vi "Main.vi"(11 "Module Admin":refnum<class "Delacor_lib_QMH_Module Admin.lvclass">) -> ()   [LabVIEW 2025, in "Auto-Process.lvlib"]
doc: "This template is based off of the Queued Message Handler design pattern and the Queued Message Handler project template that ships with LabVIEW.\n\nThe main difference is that the queue is private to this module and communication between modules is performed via Broadcast and Request events.\n\nRequest events are wrapped in public API methods and are handled in the Event Handling Loop (EHL) of this VI. Any module can register for Broadcast events sent by this module. The EHL generates messages based on user interface actions.\n\nThe Message Handling Loop (MHL) processes messages generated by the EHL, or by other messages. The messages are string values, so new messages can be added easily to the Message Cases case structure in the MHL. Each message cluster can also provide an optional value for Message Data, which is a variant that can be converted to whatever message-specific data is required.\n_____\nBased on DQMH Dev Tools: Project Template 7.1.1.1528."
uses:
  Auto-Process.lvlib
  <vilib>/Delacor/Delacor QMH/Libraries/Module Admin_class/Delacor_lib_QMH_Module Admin.lvclass
  Subvi-G/Control/XButton/button3.xctl
  <vilib>/Utility/miscctls.llb/LVPointTypeDef.ctl
  <vilib>/Utility/miscctls.llb/LVPositionTypeDef.ctl
  Module Data--cluster.ctl
  Database/Database_access.lvclass
  Do Something Argument--cluster.ctl
  <vilib>/Delacor/Delacor QMH/Libraries/Message Queue_class/Delacor_lib_QMH_Message Queue.lvclass/Delacor_lib_QMH_Message Queue.ctl
  Do Something Else Argument--cluster.ctl
  Do Something Else and Wait for Reply Argument--cluster.ctl
  Do Something Else and Wait (Reply Payload)--cluster.ctl
  Stop Argument--cluster.ctl
  <vilib>/Delacor/Delacor QMH/Libraries/Module Admin_class/Delacor_lib_QMH_Module Admin.lvclass/Delacor_lib_QMH_Module Admin.ctl
  Edit.ctl
  Origin Argument--cluster.ctl
  Init-External Argument--cluster.ctl
  Requst Execution Status Argument--cluster.ctl
  Requst Execution Status (Reply Payload)--cluster.ctl
  Receive end Argument--cluster.ctl
  <vilib>/Utility/miscctls.llb/LVBoundsTypeDef.ctl
  Database/Son-control.ctl
  <vilib>/addons/database/Auxilliary.llb/DB Tools Column Info.ctl
  <vilib>/addons/database/Auxilliary.llb/DB Tools DataTypes.ctl
  <vilib>/Delacor/Delacor QMH/Libraries/Message Queue_class/Delacor_lib_QMH_Enqueue Message (Single).vi
  <vilib>/Delacor/Delacor QMH/Libraries/Module Admin_class/Delacor_lib_QMH_Get External Launch.vi
  <vilib>/Delacor/Delacor QMH/Libraries/Message Queue_class/Delacor_lib_QMH_Enqueue Message (Array).vi
  <vilib>/Delacor/Delacor QMH/Libraries/Message Queue_class/Delacor_lib_QMH_Message Queue.lvclass
  <vilib>/addons/database/NI_Database_API.lvlib
panel:
  in  "窗口标题":string
  out "Business rule":string
  in  "Valued":string
  in  "Combo Box":string(combo)
  in  "Edit?":bool
  in  "返回主界面":bool(xcontrol)
  in  "编辑显示退表":i32[](listbox)
  in  "编辑显示进表":i32[](listbox)
  in  "编辑显示总览":i32[](listbox)
  in  "结束":bool(xcontrol)
  in  "暂停":bool(xcontrol)
  in  "开始":bool(xcontrol)
  out "logging":string
  in  "执行显示":i32[](listbox)
  in  "任务显示":i32[](listbox)
  out "error out":errorcluster
  out "X":dbl
  out "Status":string
  in  "Simulate MHL Error":bool
  in  "Simulate EHL Error":bool
  in  "Do Something Else <Replace Me>":bool
  in  "Do Something <Replace Me>":bool
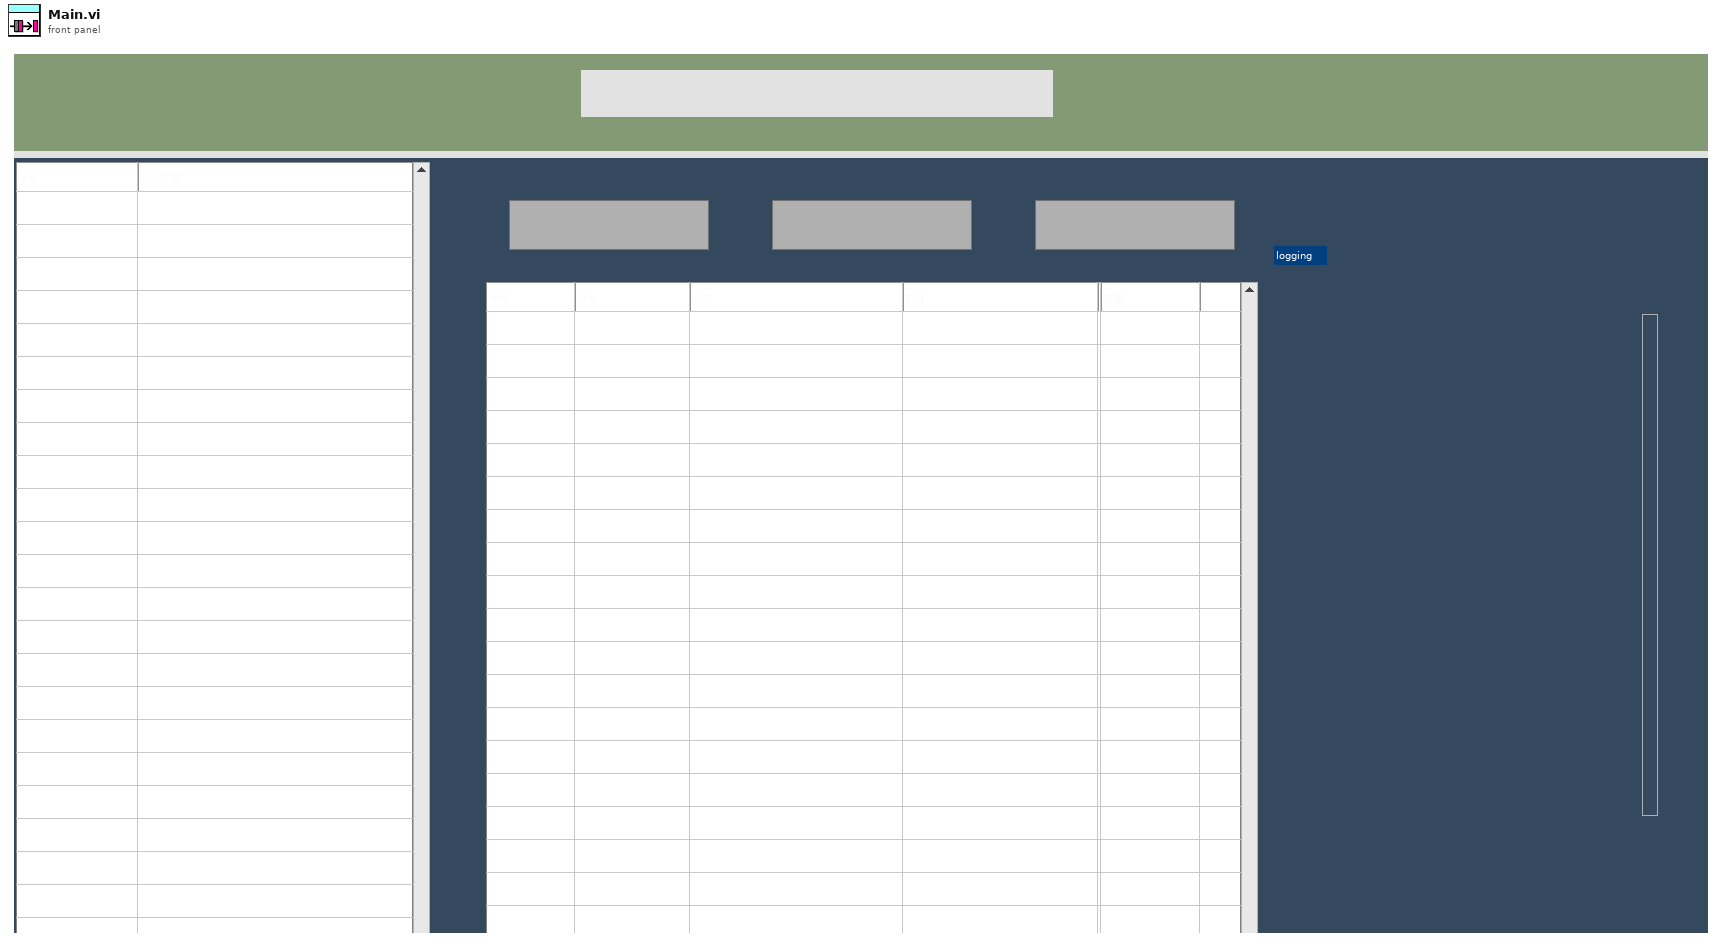
[diagram p1: front panel]
types:
  T1 = typedef "LVPositionTypeDef.ctl" = cluster{"Left":i32, "Top":i32}
  T2 = typedef "LVPointTypeDef.ctl" = cluster{"Horizontal":i16, "Vertical":i16}
  T3 = typedef "Auto-Process.lvlib/Request Events--cluster.ctl" = cluster{"Stop Module":refnum<user-event>, "Do Something":refnum<user-event>, "Do Something Else":refnum<user-event>, "Do Something Else and Wait for Reply":refnum<user-event>, "Show Panel":refnum<user-event>, "Hide Panel":refnum<user-event>, "Get Module Execution Status":refnum<user-event>, "Show Diagram":refnum<user-event>, "Origin":refnum<user-event>, "Init-External":refnum<user-event>, "Requst Execution Status":refnum<user-event>, "Receive end":refnum<user-event>, "Refursh-UI":refnum<user-event>}
  T4 = typedef "Auto-Process.lvlib/Module Data--cluster.ctl" = cluster{"Status":string, "Databas":refnum<class "Database_access.lvclass">, "总览表寄存器":string[][], "总览大小":i32[], "动作":string[][], "行为":string[], "数据类型":string[], "进表寄存器":string[][], "退表寄存器":string[][], "进退自如":u8, "选择表名":string, "New-table":string, "Old-table":string, "进退自如":bool, "行列号":cluster{"Row":i32, "Column":i32}, "项符号":i32[], "Choosed task":string[], "Remaining table":string[], "Remaining Process":string[][], "Execute Process":string[][], "暂停指令":string}
  T5 = typedef "Auto-Process.lvlib/Do Something Argument--cluster.ctl" = cluster{"Do Something Msg":string}
  T6 = typedef "Auto-Process.lvlib/Do Something Else Argument--cluster.ctl" = cluster{"Do Something Else Msg":string, "X":dbl}
  T7 = typedef "Auto-Process.lvlib/Do Something Else and Wait for Reply Argument--cluster.ctl" = cluster{"Do Something Else Msg":string, "X":dbl, "Wait Notifier":refnum<notifier>, "wait for reply":bool}
  T8 = enum32{"invalid lock state", "Not Locked", "Locked (No Password)", "Password-protected"}
  T9 = typedef "Auto-Process.lvlib/Stop Argument--cluster.ctl" = cluster{"Origin":string, "Exit via Stop Module Req?":bool, "Wait for Module to stop?":bool}
  T10 = typedef "Edit.ctl" = cluster{"单元格位置":cluster{"Row":i32, "Column":i32}, "控件引用":refnum<vi>, "进退自如":u8}
  T11 = typedef "Auto-Process.lvlib/Origin Argument--cluster.ctl" = cluster{"原点":cluster{"Horizontal":i16, "Vertical":i16}}
  T12 = typedef "Auto-Process.lvlib/Init-External Argument--cluster.ctl" = cluster{"布尔":bool}
  T13 = typedef "Auto-Process.lvlib/Requst Execution Status Argument--cluster.ctl" = cluster{"Wait Notifier":refnum<notifier>, "wait for reply":bool}
  T14 = typedef "Auto-Process.lvlib/Receive end Argument--cluster.ctl" = cluster{"Arr":string[]}
  T15 = enum32{"Invalid", "Standard", "Closed", "Hidden", "Minimized", "Maximized"}
  T16 = enum8{"Enabled", "Disabled", "Disabled and Grayed Out"}
  T17 = typedef "Auto-Process.lvlib/Do Something Else and Wait (Reply Payload)--cluster.ctl" = cluster{"Value":dbl, "error":errorcluster}
  T18 = typedef "Auto-Process.lvlib/Requst Execution Status (Reply Payload)--cluster.ctl" = cluster{"Status":enum8{"Enabled", "Disabled", "Disabled and Grayed Out"}, "error":errorcluster}
  T19 = typedef "LVBoundsTypeDef.ctl" = cluster{"Width":u32, "Height":u32}
  T20 = cluster{"退表寄存器[0]":string, "退表寄存器[1]":string, "退表寄存器[2]":string, "退表寄存器[3]":string, "退表寄存器[4]":string}
  T21 = cluster{"字符串":string, "字符串 2":string, "字符串 3":string, "字符串 4":string, "字符串 5":string}
  T22 = typedef "Son-control.ctl" = T23[]
  T23 = typedef "NI_Database_API.lvlib/DB Tools Column Info.ctl" = cluster{"column name":string, "data type":T24, "size":i32, "allow null?":bool}
  T24 = typedef "NI_Database_API.lvlib/DB Tools DataTypes.ctl" = enum16{"String", "Long (I32)", "Single (SGL)", "Double (DBL)", "Date/Time", "Binary"}
  T25 = cluster{"总览表寄存器[0]":string, "总览表寄存器[1]":string, "总览表寄存器[2]":string}
  T26 = typedef "LVPoint32TypeDef.ctl" = cluster{"Horizontal":i32, "Vertical":i32}
  T27 = typedef "LVRowAndColumnTypeDef.ctl" = cluster{"Row":i32, "Column":i32}
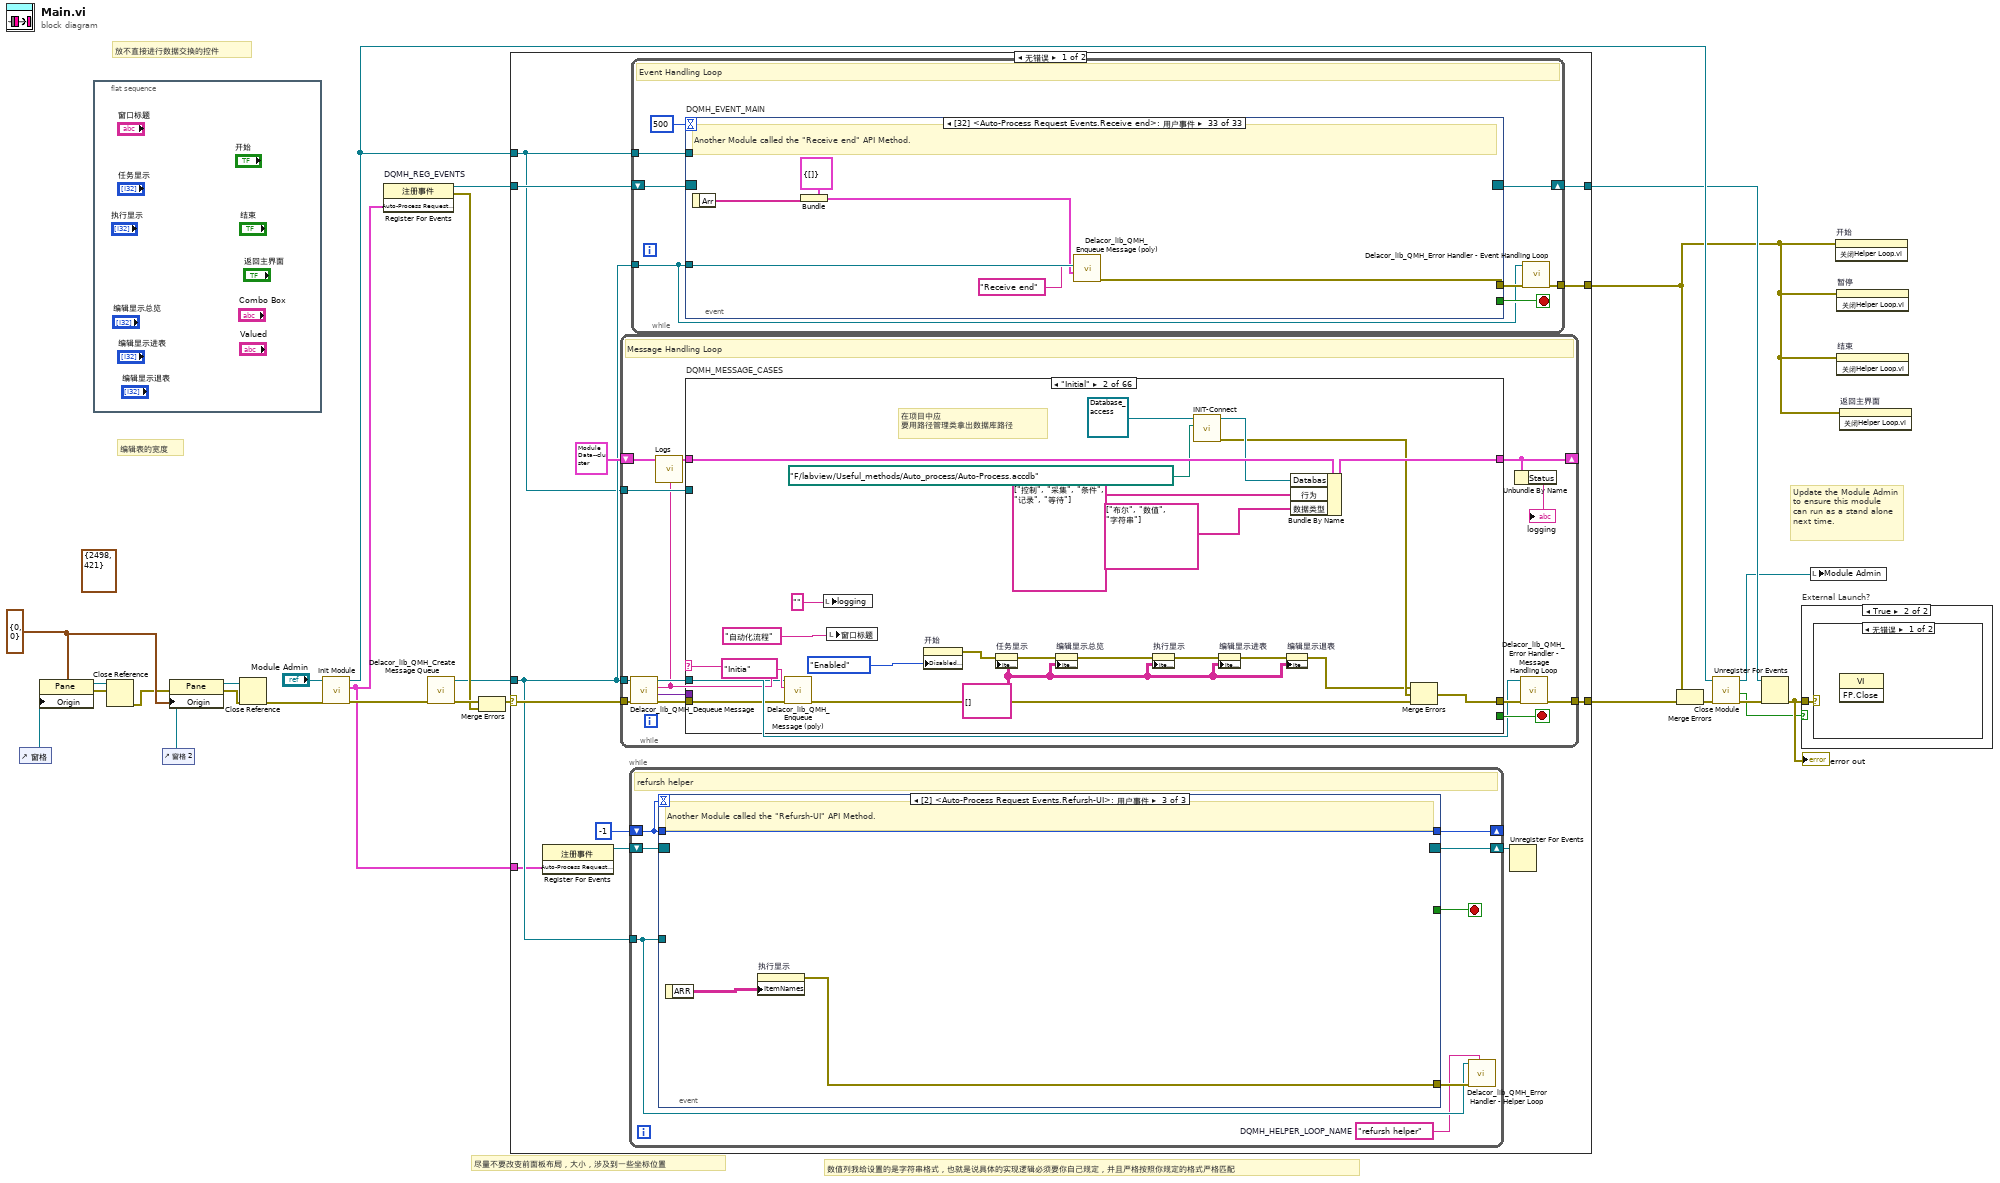
[diagram p0: block diagram]
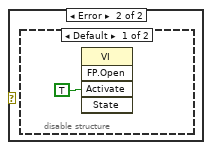
[diagram p3: hidden frame]
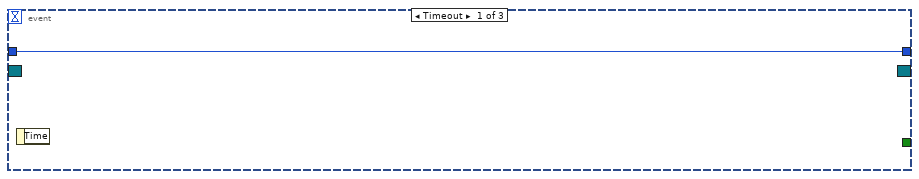
[diagram p5: hidden frame]
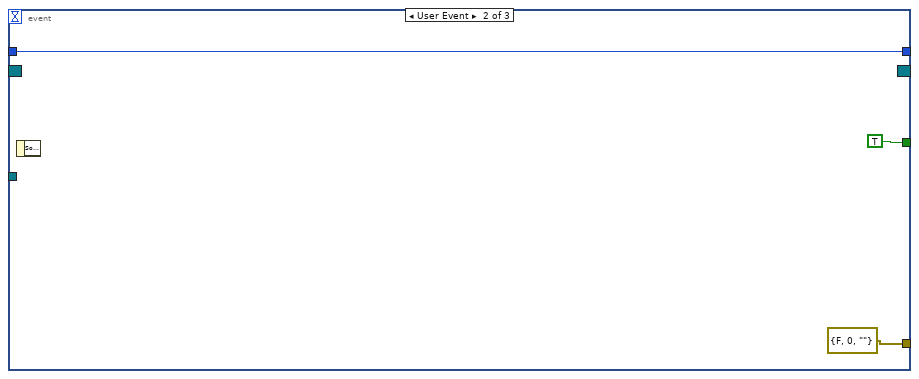
[diagram p6: hidden frame]
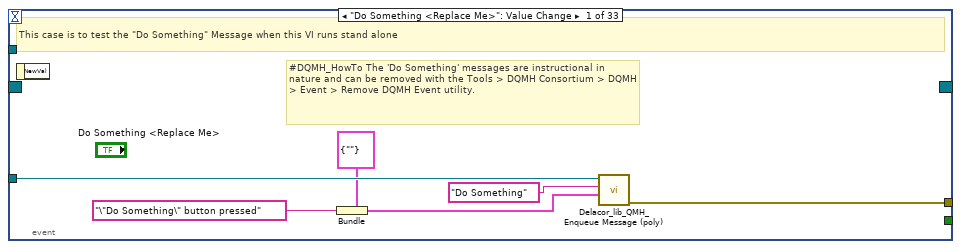
[diagram p7: hidden frame]
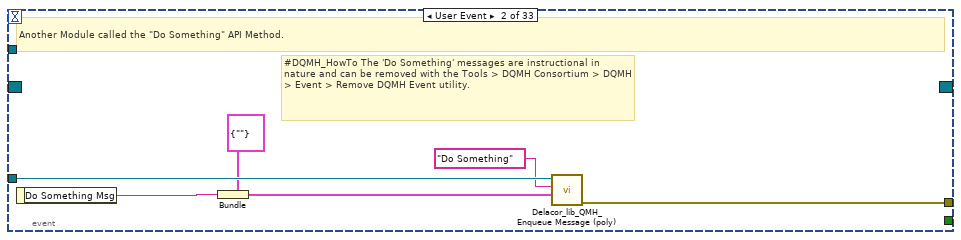
[diagram p8: hidden frame]
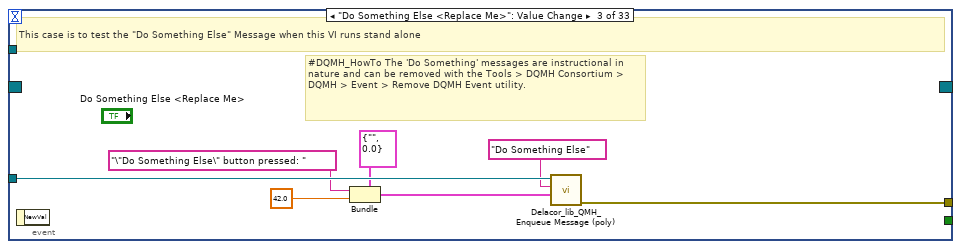
[diagram p9: hidden frame]
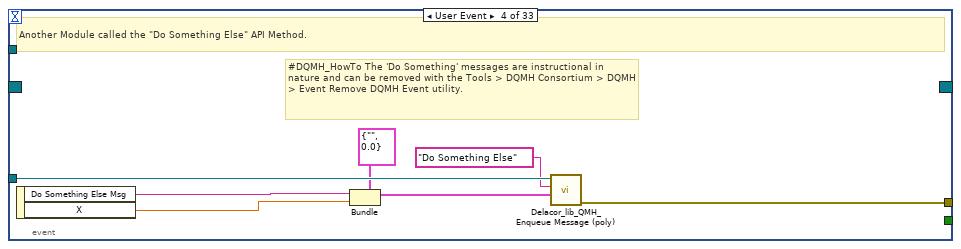
[diagram p10: hidden frame]
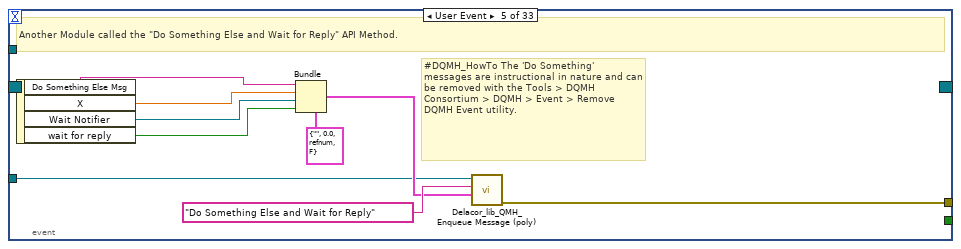
[diagram p11: hidden frame]
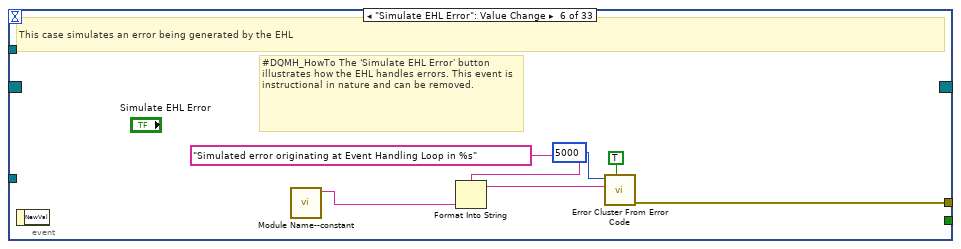
[diagram p12: hidden frame]
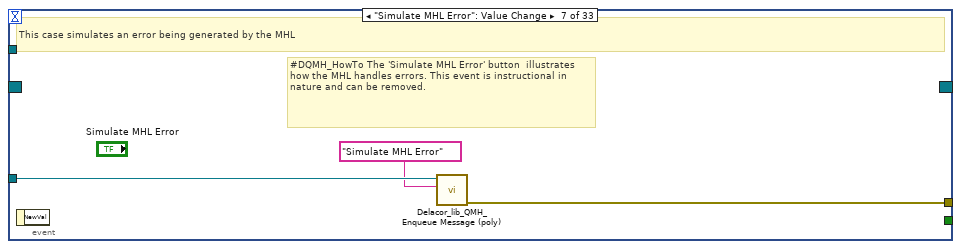
[diagram p13: hidden frame]
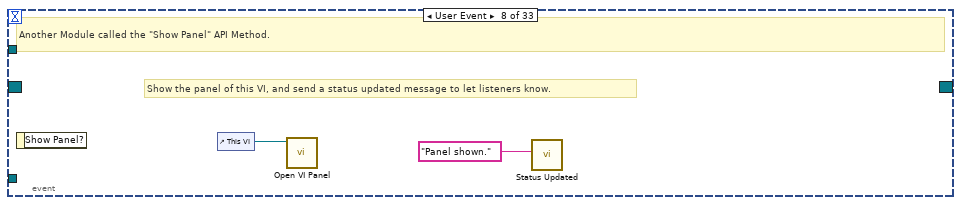
[diagram p14: hidden frame]
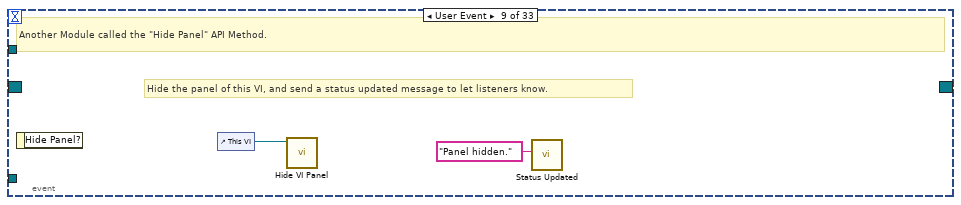
[diagram p15: hidden frame]
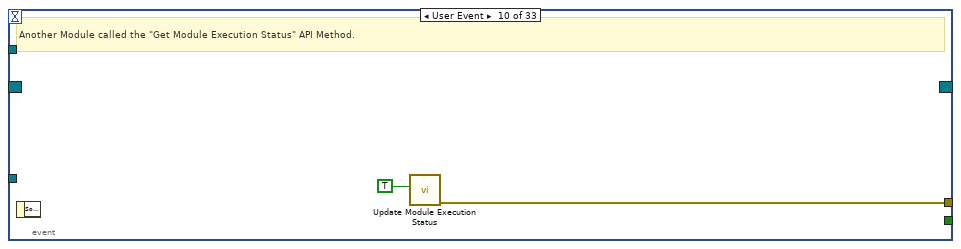
[diagram p16: hidden frame]
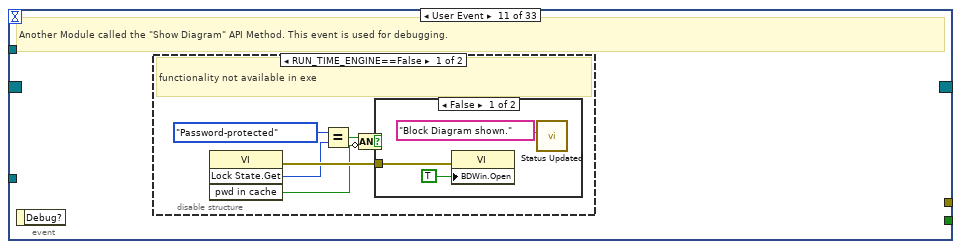
[diagram p17: hidden frame]
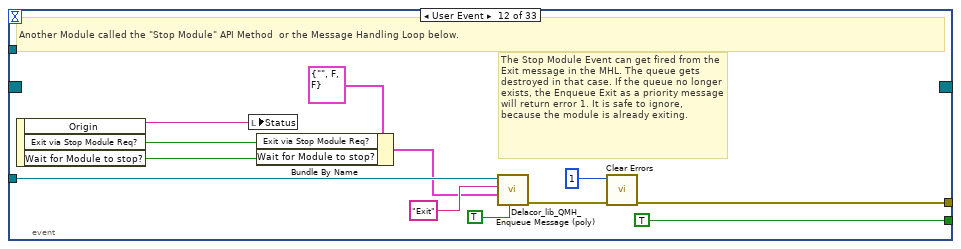
[diagram p20: hidden frame]
diagram:
  (unwired) T1 {"Left"=2498, "Top"=421} ("位置 2")
  w9 = T2 {"Horizontal"=0, "Vertical"=0} ("原点")
  # "数值列我给设置的是字符串格式，也就是说具体的实现逻辑必须要你自己规定，并且严格按照你规定的格式严格匹配"
  # "尽量不要改变前面板布局，大小，涉及到一些坐标位置"
  # "编辑表的宽度"
  # "放不直接进行数据交换的控件"
  # "Update the Module Admin to ensure this module can run as a stand alone next time."
  n1 = control-ref of="窗格"() -> (w11:refnum<vi>)
  n2 = property class="Pane"(reference=w11, "Origin"=w9) -> (reference out=w5:refnum<vi>, error out=w6:errorcluster)  [unwired: 1 in]
  n3 = flat-sequence {
    frame #0 {
    }
  }
  n4 = Close Reference(reference=w5, error in (no error)=w6) -> (error out=w4:errorcluster)
  n5 = control-ref of="窗格 2"() -> (w10:refnum<vi>)
  n6 = property class="Pane"(reference=w10, error in=w4, "Origin"=w9) -> (reference out=w7:refnum<vi>, error out=w8:errorcluster)
  n7 = Close Reference(reference=w7, error in (no error)=w8) -> (error out=w3:errorcluster)
  n8 = call "Init Module.vi"("error in"=w3, "Singleton Module Admin in"="Module Admin") -> ("error out"=w25:errorcluster, "Auto-Process Request Events"=w1:T3, "Singleton Module Admin out"=w18:refnum<class "Delacor_lib_QMH_Module Admin.lvclass">)  [unwired: 7 in]
  n9 = register-events "DQMH_REG_EVENTS"(w1) -> (reference out=w16:refnum<event-registration>, error out=w19:errorcluster)  [unwired: 2 in]
  n10 = call <vilib>:"Delacor_lib_QMH_Create Message Queue.vi"("error in"=w25) -> ("error out"=w21:errorcluster, "Message Queue"=w15:refnum<class "Delacor_lib_QMH_Message Queue.lvclass">)  [unwired: 9 in]
  n11 = Merge Errors(w21, w19) -> (w20:errorcluster)
  n12 = case shown="无错误" w20 {
    selector: w20 -> [w36 w1372]
    tunnel: [w38 w1371] -> w26
    tunnel: [w35 w1370] -> w17
    tunnel: w16 -> [w33 w1370]
    tunnel: w15 -> [w32 w1365]
    tunnel: [w37 _] -> w2
    tunnel: w18 -> [w31 w1366]
    tunnel: w1 -> [w30 _]
    frame No Error {
      n13 = register-events ("DQMH_HELPER_REGFOREVENTS")(w30) -> (reference out=w28:refnum<event-registration>)  [unwired: 2 in, 1 out]
      n14 = while {
        tunnel: w32 -> [w301]
        shift-right: [w300] -> _
        shift-left: T4 {"Status"="", "Databas"=refnum, "总览表寄存器"=[], "总览大小"=[], "动作"=[], "行为"=[], "数据类型"=[], "进表寄存器"=[], "退表寄存器"=[], "进退自如"=0, "选择表名"="", "New-table"="", "Old-table"="", "进退自如"=FALSE, "行列号"={"Row"=0, "Column"=0}, "项符号"=[], "Choosed task"=[], "Remaining table"=[], "Remaining Process"=[], "Execute Process"=[], "暂停指令"=""} ("Data Cluster") -> [w308]
        tunnel: w36 -> [w310]
        tunnel: [w304] -> w38
        tunnel: w31 -> [w305]
        stop <- w307 stop-if-true
        # "Message Handling Loop"
        n15 = call-dynamic "Delacor_lib_QMH_Dequeue Message.vi"("error in"=w310, "Message Queue in"=w301) -> ("error out"=w309:errorcluster, "Message Data"=w306:variant, "Message"=w297:string, "Message Queue out"=w302:refnum<class "Delacor_lib_QMH_Message Queue.lvclass">)  [unwired: 6 in]
        n16 = call "Logs.vi"("字符串"=w297, "Data Cluster"=w308) -> ("Module Data"=w298:T4)  [unwired: 9 in]
        n17 = case "DQMH_MESSAGE_CASES" shown="\"Initial\"" w297 {
          selector: w297 -> [_ _ _ _ _ _ _ _ _ _ _ _ _ _ _ _ _ _ _ _ _ _ _ _ _ _ _ _ _ _ _ _ _ _ _ _ _ _ _ _ _ _ _ _ _ _ _ _ _ _ _ _ _ _ _ _ _ _ _ _ _ _ _ _ _ w1360]
          tunnel: w302 -> [w315 w352 w361 w370 w385 w394 _ _ _ _ _ _ _ _ _ _ _ _ _ _ _ _ _ _ _ _ _ _ w740 w767 _ w823 _ _ _ _ w931 _ w960 w986 w1020 w1050 w1074 _ _ w1114 _ _ w1160 w1174 _ _ w1192 w1211 _ w1237 w1257 w1279 w1293 _ _ _ _ w1323 w1348 _]
          tunnel: w309 -> [w317 w351 w359 w369 w384 w393 w403 w457 w465 w474 w493 w514 w526 w531 w533 w539 w560 w569 w574 w592 w609 w635 w643 w646 w651 w658 w662 w677 w749 w776 w808 w833 w863 w878 w898 w919 w939 w943 w970 w996 w1019 w1060 w1073 w1109 w1111 w1127 w1136 w1156 w1161 w1176 w1186 w1188 w1193 w1212 w1221 w1246 w1256 w1285 w1296 w1306 w1308 w1310 w1319 w1330 w1354 w1363]
          tunnel: [w331 w348 w358 w368 w378 w400 w405 w457 w463 w473 w492 w504 w517 w530 w533 w542 w555 w564 w579 w597 w613 w638 w643 w648 w651 w660 w662 w672 w739 w766 w808 w824 w863 w878 w895 w917 w932 w942 w959 w985 w1021 w1049 w1076 w1106 w1111 w1115 w1135 w1156 w1159 w1175 w1186 w1188 w1190 w1204 w1220 w1232 w1254 w1278 w1295 w1306 w1308 w1310 w1318 w1326 w1338 w1364] -> w303
          tunnel: w298 -> [w322 w357 w366 w372 w387 w391 w411 w456 w462 w472 w489 w513 w515 w529 w532 w538 w559 w568 w581 w599 w607 w634 w642 w649 w650 w653 w661 w673 w745 w772 w807 w829 w862 w877 w901 w914 w940 w954 w972 w998 w1035 w1062 w1091 w1104 w1110 w1128 w1154 w1155 w1167 w1173 w1185 w1187 w1201 w1218 w1224 w1241 w1260 w1283 w1298 w1305 w1307 w1309 w1316 w1325 w1340 w1361]
          tunnel: [w321 w356 w363 w372 w381 w397 w411 w456 w462 w472 w489 w513 w515 w529 w532 w536 w553 w562 w571 w589 w606 w634 w642 w649 w650 w653 w661 w667 w744 w771 w807 w828 w862 w877 w883 w909 w933 w954 w965 w991 w1035 w1055 w1091 w1102 w1110 w1118 w1154 w1155 w1162 w1173 w1185 w1187 w1203 w1219 w1223 w1240 w1259 w1277 w1294 w1305 w1307 w1309 w1316 w1325 w1340 w1361] -> w300
          tunnel: [_ _ _ _ _ _ _ _ _ _ _ _ _ _ _ _ _ _ _ _ _ _ _ _ _ _ _ _ _ _ _ _ _ _ _ _ _ _ _ _ _ _ _ _ _ _ _ _ _ _ _ _ _ _ _ _ _ _ _ _ _ _ _ _ w1347 _] -> w307
          tunnel: w306 -> [_ _ _ _ _ _ _ _ w461 w469 w486 w512 w524 _ _ w540 _ _ w575 w593 w610 w636 _ _ _ _ _ w676 w748 w775 _ w832 _ _ w899 w918 w938 w948 w971 w997 _ w1061 _ _ _ w1126 w1142 _ _ _ _ _ _ _ _ w1245 _ w1284 _ _ _ _ _ w1324 w1346 _]
          tunnel: w305 -> [w323 _ _ _ _ _ _ _ _ _ _ _ _ _ _ _ _ _ _ _ _ _ _ _ _ _ _ _ _ _ _ _ _ _ _ _ _ _ _ _ _ _ _ _ _ _ _ _ _ _ _ _ _ _ _ _ _ _ _ _ _ _ _ w1322 w1341 _]
          frame "Initialize" {
            (unwired) T2 {"Horizontal"=0, "Vertical"=0} ("Origin")
            # "Initialize - Any operation that needs to be done before the module can receive messages. Synchronize Caller Events.vi will inform Start Module.vi that the module has launched and is ready to receive messages. Module Did Init.vi will broadcast that the module initialized."
            n18 = call-poly <vilib>:"Delacor_lib_QMH_Enqueue Message (poly).vi"("error in"=w317, "Message"="Initial", "Message Queue in"=w315) -> ("error out"=w316:errorcluster)  [unwired: 7 in, 1 out]
            n19 = call "Synchronize Caller Events.vi"("error in"=w316, "Singleton Module Admin in"=w323) -> ("error out"=w332:errorcluster, "Singleton Module Admin out"=w318:refnum<class "Delacor_lib_QMH_Module Admin.lvclass">)  [unwired: 8 in]
            n20 = property on="Property Node" class="Module Admin"(reference=w318) -> ("Accessors:External Launch"=w327:bool)  [unwired: 1 in, 2 out]
            n21 = Select(t=T15."Hidden" ("State"), s=w327, f=T15."Standard" ("State")) -> (s? t:f=w324:T15)
            n22 = call "Module Name--constant.vi"() -> ("Module Name"=w330:string)  [unwired: 11 in]
            n23 = property on="Property Node" class="VI"("Front Panel.Title"=w330) -> (reference out=w329:refnum<vi>, error out=w334:errorcluster)  [unwired: 2 in]
            n24 = call "Time.vi"("字符串"="Initial Message" ("Initial Message")) -> ("连接的字符串"=w312:string)  [unwired: 10 in]
            "Status" <- w312
            n25 = invoke on="Invoke Node" class="VI" method="FP.Open"(reference=w329, error in=w334, "State"=w324) -> (reference out=w328:refnum<vi>, error out=w333:errorcluster)  [unwired: 2 in, 3 out]
            n26 = Bundle By Name(cluster=w322, "Status"=w312) -> (w321:T4)
            n27 = invoke on="Invoke Node" class="VI" method="FP.Center"(reference=w328, error in=w333) -> ()  [unwired: 1 in, 3 out]
            n28 = call "Module Name--constant.vi"() -> ("Module Name"=w319:string)  [unwired: 11 in]
            n29 = call "Module Did Init.vi"("error in"=w332, "Initialized?"=TRUE, "Origin"=w319) -> ("error out"=w331:errorcluster)  [unwired: 8 in]
            "Business rule" <- "等待：数值（s）\n控制：控制量-T/F\n控制：控制量-数值" ("Business rule")
          }
          frame "Initial" {
            w346 = string[][] [] ("项名")
            # "在项目中应\n要用路径管理类拿出数据库路径"
            n30 = call-poly <vilib>:"Delacor_lib_QMH_Enqueue Message (poly).vi"("error in"=w351, "Message"="Initia", "Message Queue in"=w352) -> ("error out"=w350:errorcluster)  [unwired: 7 in, 1 out]
            n31 = local write "logging"("" ("logging")) -> ()
            n32 = local write "窗口标题"("自动化流程" ("窗口标题")) -> ()
            n33 = property on="开始" class="button3 (严格)"("DisabledEnum"=T16."Enabled" ("禁用")) -> (error out=w337:errorcluster)  [unwired: 2 in, 1 out]
            n34 = property on="任务显示" class="MCListbox (严格)"(error in=w337, "ItemNames"=w346) -> (error out=w344:errorcluster)  [unwired: 1 in, 1 out]
            n35 = property on="编辑显示总览" class="MCListbox (严格)"(error in=w344, "ItemNames"=w346) -> (error out=w343:errorcluster)  [unwired: 1 in, 1 out]
            n36 = property on="执行显示" class="MCListbox (严格)"(error in=w343, "ItemNames"=w346) -> (error out=w342:errorcluster)  [unwired: 1 in, 1 out]
            n37 = call-dynamic "INIT-Connect.vi"("database-path"=path "F:/labview/Useful_methods/Auto_process/Auto-Process.accdb", "Database_access 输入"=refnum<class "Database_access.lvclass"> refnum) -> ("error out"=w347:errorcluster, "Database_access 输出"=w349:refnum<class "Database_access.lvclass">)  [unwired: 8 in]
            n38 = property on="编辑显示进表" class="MCListbox (严格)"(error in=w342, "ItemNames"=w346) -> (error out=w345:errorcluster)  [unwired: 1 in, 1 out]
            n39 = property on="编辑显示退表" class="MCListbox (严格)"(error in=w345, "ItemNames"=w346) -> (error out=w341:errorcluster)  [unwired: 1 in, 1 out]
            n40 = Bundle By Name(cluster=w357, "Databas"=w349, "行为"=string[] ["控制", "采集", "条件", "记录", "等待"] ("窗口标题"), "数据类型"=string[] ["布尔", "数值", "字符串"] ("窗口标题")) -> (w356:T4)
            n41 = Merge Errors(w341, w347, w350) -> (w348:errorcluster)
          }
          frame "initia" {
            # "编辑好了在替换这个"
            n42 = call-poly <vilib>:"Delacor_lib_QMH_Enqueue Message (poly).vi"("error in"=w359, "Message"="Initi", "Message Queue in"=w361) -> ("error out"=w358:errorcluster)  [unwired: 7 in, 1 out]
            n43 = property on="Combo Box" class="CmbBox"("Position"=T1 {"Left"=3500, "Top"=800} ("位置")) -> ()  [unwired: 2 in, 2 out]
            n44 = property on="Valued" class="Str"("Position"=T1 {"Left"=3000, "Top"=900} ("位置")) -> ()  [unwired: 2 in, 2 out]
            n45 = Bundle By Name(cluster=w366, "动作"=string[][] [["AAA", "BBB", "CCC", "DDD"], ["EEE", "FFF", "HHH", "GGG"], ["III", "RRR", "SSS", "VVV"], ["A2", "JJ", "来来来", "ass啊"]] ("窗口标题")) -> (w363:T4)
          }
          frame "Initi" {
            n46 = call-poly <vilib>:"Delacor_lib_QMH_Enqueue Message (poly).vi"("error in"=w369, "Message"="Init", "Message Queue in"=w370) -> ("error out"=w368:errorcluster)  [unwired: 7 in, 1 out]
            n47 = property on="开始" class="button3 (严格)"("DisabledEnum"=T16."Enabled" ("禁用")) -> ()  [unwired: 2 in, 2 out]
          }
          frame "Init" {
            # "作为内部数据使用\n意义：\n尽量减少调用属性节点\n减少UI线程的调用"
            n48 = call-poly <vilib>:"Delacor_lib_QMH_Enqueue Message (poly).vi"("error in"=w384, "Message"="Ini", "Message Queue in"=w385) -> ("error out"=w383:errorcluster)  [unwired: 7 in, 1 out]
            n49 = Unbundle By Name(w387) -> ("Databas"=w386:refnum<class "Database_access.lvclass">)
            n50 = call-dynamic "Read_database.vi"("table"="总览", "Database_access 输入"=w386) -> ("error out"=w379:errorcluster, "data"=w380:variant[][])  [unwired: 7 in, 1 out]
            n51 = call "StringArr-type"("error in (no error)"=w379, "database variant"=w380) -> ("error out"=w377:errorcluster, "data"=w373:string[][])  [unwired: 8 in]
            n52 = property on="编辑显示总览" class="MCListbox (严格)"("ItemNames"=w373) -> (error out=w376:errorcluster)  [unwired: 2 in, 1 out]
            n53 = property on="任务显示" class="MCListbox (严格)"("ItemNames"=w373) -> (error out=w375:errorcluster)  [unwired: 2 in, 1 out]
            n54 = Array Size(array=w373) -> (size(s)=w374:i32[])
            n55 = Bundle By Name(cluster=w387, "总览表寄存器"=w373, "总览大小"=w374) -> (w381:T4)
            n56 = Merge Errors(w375, w376, w377, w383) -> (w378:errorcluster)
          }
          frame "Ini" {
            n57 = call-poly <vilib>:"Delacor_lib_QMH_Enqueue Message (poly).vi"("error in"=w393, "Message"="In", "Message Queue in"=w394) -> ("error out"=w392:errorcluster)  [unwired: 7 in, 1 out]
            n58 = call "Logs.vi"("字符串"="资源加载中......", "Data Cluster"=w391) -> ("Module Data"=w390:T4)  [unwired: 9 in]
            n59 = Unbundle By Name(w391) -> ("总览大小"=w398:i32[])
            n60 = Index Array(array=w398) -> (element=w401:i32)  [unwired: 1 in]
            n61 = Initialize Array(37, w401) -> (w396:i32[])
            n62 = property on="任务显示" class="MCListbox (严格)"("ItemSyms"=w396) -> (error out=w399:errorcluster)  [unwired: 2 in, 1 out]
            n63 = Merge Errors(w399, w392) -> (w400:errorcluster)
            n64 = Bundle By Name(cluster=w390, "项符号"=w396) -> (w397:T4)
          }
          frame "In" {
            w406 = enum16{"风格一", "风格二", "风格三", "风格四"}[] [enum."风格一", enum."风格二", enum."风格三", enum."风格四"] items=["风格一", "风格二", "风格三", "风格四"] ("动效风格")
            # "这里有点耗时\n需要约1s"
            n65 = control-ref of="窗格 2"() -> (w410:refnum<vi>)
            n66 = for {
              tunnel: w410 -> [w417]
              tunnel: string[] ["开始", "暂停", "结束", "返回"] ("布尔文本") -> [w416] mode=indexing
              tunnel: u32 16777225 -> [w415]
              tunnel: u32 35 ("布尔文本字号") -> [w414]
              tunnel: w406 -> [w413] mode=indexing
              tunnel: [w412] -> w404 mode=indexing
              i -> [w418]
              n67 = case shown="0" w418 {
                tunnel: w417 -> [_ w427 w437 w446 w455]
                tunnel: w416 -> [_ w426 w436 w445 w454]
                tunnel: w415 -> [_ w425 w435 w444 w453]
                tunnel: w414 -> [_ w424 w434 w443 w452]
                tunnel: w413 -> [_ w423 w433 w442 w451]
                tunnel: [_ w420 w430 w439 w448] -> w412
                frame Default {
                }
                frame 0 {
                  n68 = control-ref of="开始"() -> (w419:refnum<vi>)
                  n69 = property on="属性节点" class="button3 (严格)"(reference=w419, "窗格引用"=w427, "布尔文本"=w426, "布尔文本颜色"=w425, "布尔文本字号"=w424, "动效风格"=w423) -> (reference out=w421:refnum<vi>, error out=w422:errorcluster)  [unwired: 1 in]
                  n70 = invoke on="调用节点" class="button3 (严格)" method="启动helper loop.vi"(reference=w421, error in=w422) -> (error out=w420:errorcluster)  [unwired: 1 in, 2 out]
                }
                frame 1 {
                  n71 = control-ref of="暂停"() -> (w429:refnum<vi>)
                  n72 = property on="属性节点" class="button3 (严格)"(reference=w429, "窗格引用"=w437, "布尔文本"=w436, "布尔文本颜色"=w435, "布尔文本字号"=w434, "动效风格"=w433, "Value"=FALSE ("值")) -> (reference out=w431:refnum<vi>, error out=w432:errorcluster)  [unwired: 1 in]
                  n73 = invoke on="调用节点" class="button3 (严格)" method="启动helper loop.vi"(reference=w431, error in=w432) -> (error out=w430:errorcluster)  [unwired: 1 in, 2 out]
                }
                frame 2 {
                  n74 = control-ref of="结束"() -> (w438:refnum<vi>)
                  n75 = property on="属性节点" class="button3 (严格)"(reference=w438, "窗格引用"=w446, "布尔文本"=w445, "布尔文本颜色"=w444, "布尔文本字号"=w443, "动效风格"=w442) -> (reference out=w440:refnum<vi>, error out=w441:errorcluster)  [unwired: 1 in]
                  n76 = invoke on="调用节点" class="button3 (严格)" method="启动helper loop.vi"(reference=w440, error in=w441) -> (error out=w439:errorcluster)  [unwired: 1 in, 2 out]
                }
                frame 3 {
                  n77 = control-ref of="返回主界面"() -> (w447:refnum<vi>)
                  n78 = property on="属性节点" class="button3 (严格)"(reference=w447, "窗格引用"=w455, "布尔文本"=w454, "布尔文本颜色"=w453, "布尔文本字号"=w452, "动效风格"=w451) -> (reference out=w449:refnum<vi>, error out=w450:errorcluster)  [unwired: 1 in]
                  n79 = invoke on="调用节点" class="button3 (严格)" method="启动helper loop.vi"(reference=w449, error in=w450) -> (error out=w448:errorcluster)  [unwired: 1 in, 2 out]
                }
              }
            }
            n80 = Merge Errors(w404, w403) -> (w405:errorcluster)
          }
          frame "---Module Specific---" {
            # "Separator -- The following cases handle messages specific to this Module."
          }
          frame "Do Something" {
            # "Do Something - Replace this message with functionality for your own application. Note that this message also fires the \"Did Something\" broadcast event."
            n81 = Variant To Data(error in=w465, type=T5 {"Do Something Msg"=""} ("Do Something Argument"), Variant=w461) -> (data=w460:T5, error out=w464:errorcluster)
            n82 = Unbundle By Name(w460) -> ("Do Something Msg"=w458:string)
            n83 = call "Did Something.vi"("error in"=w464, "Did Something Msg"=w458) -> ("error out"=w463:errorcluster)  [unwired: 9 in]
            n84 = call "Status Updated.vi"("Status"=w458) -> ()  [unwired: 10 in, 1 out]
            n85 = local write "Status"(w458) -> ()
          }
          frame "Do Something Else" {
            # "Do Something Else - Replace this message with functionality for your own application."
            n86 = Variant To Data(error in=w474, type=T6 {"Do Something Else Msg"="", "X"=0.0} ("Do Something Else Argument"), Variant=w469) -> (data=w470:T6, error out=w473:errorcluster)
            n87 = Unbundle By Name(w470) -> ("Do Something Else Msg"=w468:string, "X"=w467:dbl)
            "X" <- w467
            n88 = Format Into String(initial string=w468, w467) -> (resulting string=w466:string)  [unwired: 2 in, 1 out]
            n89 = local write "Status"(w466) -> ()
            n90 = call "Status Updated.vi"("Status"=w466) -> ()  [unwired: 10 in, 1 out]
          }
          frame "Do Something Else and Wait for Reply" {
            w481 = "X(%.2f)+Offset(%.2f)=%.2f"  # status message format string
            # "#DQMH_HowTo The 'Do Something' messages are instructional in nature and can be removed."
            # "Send back X with a random offset"
            # "Do Something Else and Wait for Reply - Replace this message with functionality for your own application. Note that this message must fire a notifier to let callers know it has finished execution, and it returns an error if the 'Value' is negative."
            n91 = Variant To Data(error in=w493, type=T7 {"Do Something Else Msg"="", "X"=0.0, "Wait Notifier"=refnum, "wait for reply"=FALSE} ("Do Something Else and Wait for Reply Argument"), Variant=w486) -> (data=w487:T7, error out=w491:errorcluster)
            n92 = Unbundle By Name(w487) -> ("Wait Notifier"=w475:refnum<notifier>, "Do Something Else Msg"=w485:string, "X"=w482:dbl, "wait for reply"=w478:bool)
            n93 = Random Number (0-1)() -> (number: 0 to 1=w483:dbl)
            n94 = Add(x=w483, y=w482) -> (x+y=w477:dbl)
            n95 = Less Than 0?(x=w477) -> (x < 0?=w480:bool)
            n96 = local write "X"(w482) -> ()
            n97 = case shown="True" w480 {
              tunnel: [_ w503] -> w490
              frame False {
              }
              frame True {
                n98 = call <vilib>:"Error Cluster From Error Code.vi"("show call chain? (False)"=TRUE, "error message (\"\")"="The 'Something Else and Wait for Reply' message generated a negative number, which is considered an error condition.", "error code (0)"=5000) -> ("error out"=w503:errorcluster)  [unwired: 6 in]
              }
            }
            n99 = Format Into String(format string=w481, initial string=w485, w482, w483, w477) -> (resulting string=w479:string)  [unwired: 1 in, 1 out]
            n100 = Bundle By Name(cluster=T17 {"Value"=0.0, "error"={"status"=FALSE, "code"=0, "source"=""}} ("notification"), "error"=w490, "Value"=w477) -> (w476:T17)
            n101 = local write "Status"(w479) -> ()
            n102 = call "Status Updated.vi"("Status"=w479) -> ()  [unwired: 10 in, 1 out]
            n103 = case shown="True" w478 {
              tunnel: w476 -> [_ w496]
              tunnel: w475 -> [_ w495]
              frame False {
              }
              frame True {
                # "Simulate an operation that requires a wait."
                n104 = flat-sequence {
                  tunnel: w496 -> [w499]
                  tunnel: w495 -> [w498]
                  tunnel: w494 -> [_]
                  frame #0 {
                    n105 = Send Notification(notification=w499, notifier=w498) -> ()  [unwired: 1 in, 2 out]
                  }
                }
                n106 = Wait (ms)(milliseconds to wait=u32 1000) -> (millisecond timer value=w494:u32)
              }
            }
            n107 = Merge Errors(w491, w490) -> (w492:errorcluster)
          }
          frame "Origin" {
            # "改变前面版位置"
            n108 = Variant To Data(error in=w514, type=T11 {"原点"={"Horizontal"=0, "Vertical"=0}} ("Origin Argument"), Variant=w512) -> (data=w510:T11, error out=w505:errorcluster)
            n109 = Unbundle By Name(w510) -> ("原点"=w507:cluster{"Horizontal":i16, "Vertical":i16})
            n110 = control-ref of="窗格 2"() -> (w506:refnum<vi>)
            n111 = property class="Pane"(reference=w506, error in=w505, "Origin"=w507) -> (reference out=w508:refnum<vi>, error out=w509:errorcluster)
            n112 = Close Reference(reference=w508, error in (no error)=w509) -> (error out=w504:errorcluster)
          }
          frame "Requst Execution Status" {
            # "外部询问执行状态"
            n113 = Variant To Data(error in=w526, type=T13 {"Wait Notifier"=refnum, "wait for reply"=FALSE} ("Requst Execution Status Argument"), Variant=w524) -> (data=w522:T13, error out=w525:errorcluster)
            n114 = Unbundle By Name(w522) -> ("Wait Notifier"=w521:refnum<notifier>, "wait for reply"=w520:bool)
            n115 = property on="开始" class="button3 (严格)"() -> ("DisabledEnum"=w516:T16)  [unwired: 2 in, 2 out]
            n116 = Merge Errors(w525) -> (w517:errorcluster)
            n117 = Bundle By Name(cluster=T18 {"Status"=enum."Enabled", "error"={"status"=FALSE, "code"=0, "source"=""}} ("Requst Execution Status (Reply Payload)"), "Status"=w516) -> (w519:T18)
            n118 = case "DQMH_FIRE_NOTIFIER" shown="True" w520 {
              tunnel: w521 -> [_ w528]
              tunnel: w519 -> [_ w527]
              frame False {
              }
              frame True {
                n119 = Send Notification(notification=w527, notifier=w528) -> ()  [unwired: 1 in, 2 out]
              }
            }
          }
          frame "---Copy This Frame---" {
            # "Duplicate this frame when creating new messages.  Change this comment in the duplicated frame to describe this message."
            n120 = Merge Errors(w531) -> (w530:errorcluster)
          }
          frame "-----------------A-----------------" {
          }
          frame "Select" {
            # "点一个改一个，重复点取反，"
            n121 = Variant To Data(error in=w539, type=0 ("Row"), Variant=w540) -> (data=w537:i32, error out=w534:errorcluster)
            n122 = in-place {
              in-place-border: w537 -> [w545]
              in-place-border: [w543] -> w535
              n123 = in-place-cluster #1(w538) -> ("项符号"=w546:i32[])
              n124 = in-place {
                w550 = 37 ("x")
                n125 = in-place-array #2(w546, w545) -> (w547:i32)
                n126 = Equal?(x=w550, y=w547) -> (x = y?=w551:bool)
                n127 = Select(t=38, s=w551, f=w550) -> (s? t:f=w548:i32)
                n128 = in-place-array #2(w548) -> (w544:i32[])  [unwired: 1 out]
              }
              n129 = property on="任务显示" class="MCListbox (严格)"("ItemSyms"=w544) -> (error out=w543:errorcluster)  [unwired: 2 in, 1 out]
              n130 = in-place-cluster #1("项符号"=w544) -> (w536:T4)
            }
            n131 = Merge Errors(w535, w534) -> (w542:errorcluster)
          }
          frame "Select All" {
            n132 = Unbundle By Name(w559) -> ("总览大小"=w558:i32[])
            n133 = Index Array(array=w558) -> (element=w557:i32)  [unwired: 1 in]
            n134 = Initialize Array(38, w557) -> (w552:i32[])
            n135 = property on="任务显示" class="MCListbox (严格)"("ItemSyms"=w552) -> (error out=w554:errorcluster)  [unwired: 2 in, 1 out]
            n136 = Bundle By Name(cluster=w559, "项符号"=w552) -> (w553:T4)
            n137 = Merge Errors(w554, w560) -> (w555:errorcluster)
          }
          frame "Deselect All" {
            n138 = Unbundle By Name(w568) -> ("总览大小"=w567:i32[])
            n139 = Index Array(array=w567) -> (element=w566:i32)  [unwired: 1 in]
            n140 = Initialize Array(37, w566) -> (w561:i32[])
            n141 = property on="任务显示" class="MCListbox (严格)"("ItemSyms"=w561) -> (error out=w563:errorcluster)  [unwired: 2 in, 1 out]
            n142 = Bundle By Name(cluster=w568, "项符号"=w561) -> (w562:T4)
            n143 = Merge Errors(w563, w569) -> (w564:errorcluster)
          }
          frame "Start From Here" {
            n144 = Variant To Data(error in=w574, type=0 ("Row"), Variant=w575) -> (data=w572:i32, error out=w573:errorcluster)
            n145 = Unbundle By Name(w581) -> ("总览大小"=w580:i32[])
            n146 = Index Array(array=w580) -> (element=w577:i32)  [unwired: 1 in]
            n147 = for {
              N: w577 -> [_]
              tunnel: w572 -> [w586]
              tunnel: [w582] -> w570 mode=indexing
              i -> [w587]
              n148 = Greater Or Equal?(x=w587, y=w586) -> (x >= y?=w585:bool)
              n149 = Select(t=38 ("FocusRow"), s=w585, f=37 ("FocusRow")) -> (s? t:f=w582:i32)
            }
            n150 = property on="任务显示" class="MCListbox (严格)"("ItemSyms"=w570) -> (error out=w578:errorcluster)  [unwired: 2 in, 1 out]
            n151 = Bundle By Name(cluster=w581, "项符号"=w570) -> (w571:T4)
            n152 = Merge Errors(w578, w573) -> (w579:errorcluster)
          }
          frame "End At Here" {
            n153 = Variant To Data(error in=w592, type=0 ("Row"), Variant=w593) -> (data=w590:i32, error out=w591:errorcluster)
            n154 = Unbundle By Name(w599) -> ("总览大小"=w598:i32[])
            n155 = Index Array(array=w598) -> (element=w595:i32)  [unwired: 1 in]
            n156 = for {
              N: w595 -> [_]
              tunnel: w590 -> [w604]
              tunnel: [w600] -> w588 mode=indexing
              i -> [w605]
              n157 = Less Or Equal?(x=w605, y=w604) -> (x <= y?=w603:bool)
              n158 = Select(t=38 ("FocusRow"), s=w603, f=37 ("FocusRow")) -> (s? t:f=w600:i32)
            }
            n159 = property on="任务显示" class="MCListbox (严格)"("ItemSyms"=w588) -> (error out=w596:errorcluster)  [unwired: 2 in, 1 out]
            n160 = Bundle By Name(cluster=w599, "项符号"=w588) -> (w589:T4)
            n161 = Merge Errors(w596, w591) -> (w597:errorcluster)
          }
          frame "Invert Selection" {
            # "反选"
            n162 = Variant To Data(error in=w609, type=0 ("Row"), Variant=w610) -> (error out=w608:errorcluster)  [unwired: 1 out]
            n163 = in-place {
              in-place-border: [w616] -> w612
              n164 = in-place-cluster #3(w607) -> ("项符号"=w615:i32[])
              n165 = for {
                tunnel: [w619] -> w614 mode=indexing
                tunnel: w615 -> [w617] mode=indexing
                w618 = 37 ("FocusRow")
                n166 = Equal?(x=w617, y=w618) -> (x = y?=w621:bool)
                n167 = Select(t=38 ("FocusRow"), s=w621, f=w618) -> (s? t:f=w619:i32)
              }
              n168 = property on="任务显示" class="MCListbox (严格)"("ItemSyms"=w614) -> (error out=w616:errorcluster)  [unwired: 2 in, 1 out]
              n169 = in-place-cluster #3("项符号"=w614) -> (w606:T4)
            }
            n170 = Merge Errors(w612, w608) -> (w613:errorcluster)
          }
          frame "Show" {
            # "拿出表名"
            # "根据点的行去数据库拿对应的表，点到空白则不拿了\n只拿进表\n1：进    2：退"
            n171 = Variant To Data(error in=w635, type=0 ("Row"), Variant=w636) -> (data=w632:i32, error out=w627:errorcluster)
            n172 = Unbundle By Name(w634) -> ("Databas"=w630:refnum<class "Database_access.lvclass">, "总览表寄存器"=w633:string[][])
            n173 = Index Array(array=w633, index (row) #1=w632, index (col) #1=1 ("禁用的索引 (列)")) -> (element #1=w622:string, element #2=w623:string)  [unwired: 2 in]
            n174 = call "Indicator-string.vi"("字符串"=w623) -> ("进表名"=w624:string)  [unwired: 8 in, 2 out]
            n175 = call-dynamic "Read_database.vi"("table"=w624, "Database_access 输入"=w630) -> ("error out"=w625:errorcluster, "data"=w629:variant[][])  [unwired: 7 in, 1 out]
            n176 = case shown="错误" w625 {
              tunnel: w622 -> [_ w640]
              frame No Error {
              }
              frame Error {
                n177 = Format Into String(format string="数据库无%S项\n请检查" ("字符串"), w640) -> (resulting string=w639:string)  [unwired: 2 in, 1 out]
                n178 = One Button Dialog(message=w639) -> ()  [unwired: 1 in, 1 out]
              }
            }
            n179 = call "StringArr-type"("database variant"=w629) -> ("data"=w628:string[][])  [unwired: 9 in, 1 out]
            n180 = property on="执行显示" class="MCListbox (严格)"("ItemNames"=w628) -> (error out=w626:errorcluster)  [unwired: 2 in, 1 out]
            n181 = Merge Errors(w626, w627) -> (w638:errorcluster)
          }
          frame "-----------------B-----------------" {
          }
          frame "Edit" {
            n182 = local write "窗口标题"("自动工步编辑" ("窗口标题")) -> ()
            n183 = call "Origin.vi"("error in"=w646, "原点"=cluster{"Horizontal":i16, "Vertical":i16} {"Horizontal"=2000, "Vertical"=0}) -> ("error out"=w645:errorcluster)  [unwired: 9 in]
            n184 = Merge Errors(w645) -> (w648:errorcluster)
          }
          frame "Cancel" {
          }
          frame "Return" {
            n185 = Unbundle By Name(w653) -> ("总览表寄存器"=w652:string[][])
            n186 = property on="任务显示" class="MCListbox (严格)"("ItemNames"=w652) -> ()  [unwired: 2 in, 2 out]
            n187 = property on="Combo Box" class="CmbBox"("Position"=T1 {"Left"=3000, "Top"=800} ("位置")) -> ()  [unwired: 2 in, 2 out]
            n188 = call "Origin.vi"("error in"=w658, "原点"=cluster{"Horizontal":i16, "Vertical":i16} {"Horizontal"=0, "Vertical"=0}) -> ("error out"=w657:errorcluster)  [unwired: 9 in]
            n189 = local write "窗口标题"("自动化流程" ("窗口标题")) -> ()
            n190 = property on="Valued" class="Str"("Position"=T1 {"Left"=3000, "Top"=900} ("位置")) -> ()  [unwired: 2 in, 2 out]
            n191 = Merge Errors(w657) -> (w660:errorcluster)
          }
          frame "-----------------C-----------------" {
          }
          frame "Edit-1/2" {
            # "这里的属性节点由人点击触发\n所以对系统的负载等于零"
            # "单元格长宽"
            n192 = Variant To Data(error in=w677, type=T10 {"单元格位置"={"Row"=0, "Column"=0}, "控件引用"=refnum, "进退自如"=0}, Variant=w676) -> (data=w674:T10, error out=w672:errorcluster)
            n193 = Unbundle By Name(w674) -> ("单元格位置.Column"=w669:i32, "控件引用"=w668:refnum<vi>, "单元格位置"=w663:cluster{"Row":i32, "Column":i32}, "进退自如"=w666:u8)
            n194 = property on="属性节点" class="MCListbox (严格)"(reference=w668, "ActiveCell"=w663) -> ("ActiveCellPos"=w665:T1)  [unwired: 1 in, 2 out]
            n195 = Index Array(array=T19[] [{"Width"=87, "Height"=31}, {"Width"=113, "Height"=31}, {"Width"=211, "Height"=31}, {"Width"=193, "Height"=31}, {"Width"=98, "Height"=31}, {"Width"=97, "Height"=31}] ("数组"), index=w669) -> (element=w670:T19)
            n196 = call "1or2.vi"("活动单元格:位置"=w665) -> ("1/2"=w664:bool)  [unwired: 10 in]
            n197 = Bundle By Name(cluster=w673, "进退自如"=w666, "进退自如"=w664, "行列号"=w663) -> (w667:T4)
            n198 = case shown="2" w669 {
              tunnel: w673 -> [_ w685 w698 w719 w731]
              tunnel: w670 -> [_ w683 w697 w714 w729]
              tunnel: w665 -> [_ w682 w696 w713 w728]
              tunnel: w666 -> [_ w680 w695 w718 w724]
              tunnel: w663 -> [_ w678 w694 w716 w725]
              frame 0, Default {
              }
              frame 1 {
                n199 = case shown="1, 默认" w680 {
                  tunnel: w685 -> [w688 w691]
                  tunnel: [w687 w690] -> w684
                  tunnel: [w686 w689] -> w679
                  frame 1, Default {
                    n200 = Unbundle By Name(w688) -> ("行为"=w687:string[], "进表寄存器"=w686:string[][])
                  }
                  frame 2 {
                    n201 = Unbundle By Name(w691) -> ("行为"=w690:string[], "退表寄存器"=w689:string[][])
                  }
                }
                n202 = call "Valued.vi"("单元格位置"=w678, "数组"=w679) -> ("元素"=w681:string)  [unwired: 9 in]
                n203 = property on="Combo Box" class="CmbBox"("Strings[]"=w684, "Size"=w683, "Position"=w682, "Value"=w681) -> ()  [unwired: 2 in, 2 out]
              }
              frame 2 {
                n204 = case shown="2" w695 {
                  tunnel: w698 -> [w705 w712]
                  tunnel: w694 -> [w701 w708]
                  tunnel: [w700 w707] -> w692
                  tunnel: [w699 w706] -> w693
                  frame 1, Default {
                    n205 = Unbundle By Name(w705) -> ("动作"=w704:string[][], "行为"=w703:string[], "进表寄存器"=w702:string[][])
                    n206 = call "Match.vi"("单元格位置"=w701, "数据"=w702, "行为"=w703, "动作"=w704) -> ("元素"=w700:string, "子数组"=w699:string[])  [unwired: 6 in]
                  }
                  frame 2 {
                    n207 = Unbundle By Name(w712) -> ("动作"=w711:string[][], "行为"=w710:string[], "退表寄存器"=w709:string[][])
                    n208 = call "Match.vi"("单元格位置"=w708, "数据"=w709, "行为"=w710, "动作"=w711) -> ("元素"=w707:string, "子数组"=w706:string[])  [unwired: 6 in]
                  }
                }
                n209 = property on="Combo Box" class="CmbBox"("Strings[]"=w693, "Size"=w697, "Position"=w696, "Value"=w692) -> ()  [unwired: 2 in, 2 out]
              }
              frame 3 {
                n210 = case shown="2" w718 {
                  tunnel: w719 -> [w721 w723]
                  tunnel: [w720 w722] -> w717
                  frame 1, Default {
                    n211 = Unbundle By Name(w721) -> ("进表寄存器"=w720:string[][])
                  }
                  frame 2 {
                    n212 = Unbundle By Name(w723) -> ("退表寄存器"=w722:string[][])
                  }
                }
                n213 = call "Valued.vi"("单元格位置"=w716, "数组"=w717) -> ("元素"=w715:string)  [unwired: 9 in]
                n214 = property on="Valued" class="Str"("Value"=w715, "Size"=w714, "Position"=w713) -> ()  [unwired: 2 in, 2 out]
              }
              frame 4 {
                n215 = case shown="2" w724 {
                  tunnel: w731 -> [w734 w737]
                  tunnel: [w733 w736] -> w730
                  tunnel: [w732 w735] -> w726
                  frame 1, Default {
                    n216 = Unbundle By Name(w734) -> ("数据类型"=w733:string[], "进表寄存器"=w732:string[][])
                  }
                  frame 2 {
                    n217 = Unbundle By Name(w737) -> ("数据类型"=w736:string[], "退表寄存器"=w735:string[][])
                  }
                }
                n218 = call "Valued.vi"("单元格位置"=w725, "数组"=w726) -> ("元素"=w727:string)  [unwired: 9 in]
                n219 = property on="Combo Box" class="CmbBox"("Strings[]"=w730, "Size"=w729, "Position"=w728, "Value"=w727) -> ()  [unwired: 2 in, 2 out]
              }
            }
          }
          frame "Add_Up" {
            n220 = Variant To Data(error in=w749, type=cluster{"Row":i32, "进退自如":i32} {"Row"=0, "进退自如"=2}, Variant=w748) -> (data=w746:cluster{"Row":i32, "进退自如":i32}, error out=w741:errorcluster)
            n221 = Unbundle By Name(w746) -> ("进退自如"=w743:i32, "Row"=w742:i32)
            n222 = in-place {
              in-place-border: w743 -> [w756]
              in-place-border: w743 -> [w754]
              in-place-border: w742 -> [w750]
              n223 = in-place-cluster #4(w745) -> ("进表寄存器"=w755:string[][], "退表寄存器"=w753:string[][])  [unwired: 1 out]
              n224 = case shown="2" w754 {
                tunnel: w755 -> [w759 w764]
                tunnel: w753 -> [w760 w763]
                tunnel: [w760 w761] -> w752
                tunnel: [w757 w764] -> w751
                tunnel: w750 -> [w758 w762]
                frame 1, Default {
                  n225 = call "Add-data.vi"("Indix"=w758, "数组"=w759) -> ("输出数组"=w757:string[][])  [unwired: 9 in]
                  n226 = property on="编辑显示进表" class="多列列表框 (严格)"("ItemNames"=w757) -> ()  [unwired: 2 in, 2 out]
                }
                frame 2 {
                  n227 = call "Add-data.vi"("Indix"=w762, "数组"=w763) -> ("输出数组"=w761:string[][])  [unwired: 9 in]
                  n228 = property on="编辑显示退表" class="多列列表框 (严格)"("ItemNames"=w761) -> ()  [unwired: 2 in, 2 out]
                }
              }
              n229 = in-place-cluster #4("进退自如"=w756, "进表寄存器"=w751, "退表寄存器"=w752) -> (w744:T4)
            }
            n230 = call-poly <vilib>:"Delacor_lib_QMH_Enqueue Message (poly).vi"("error in"=w741, "Message"="Add-Edit-data", "Message Queue in"=w740) -> ("error out"=w739:errorcluster)  [unwired: 7 in, 1 out]
          }
          frame "Add_Down" {
            n231 = Variant To Data(error in=w776, type=cluster{"Row":i32, "进退自如":i32} {"Row"=0, "进退自如"=2}, Variant=w775) -> (data=w773:cluster{"Row":i32, "进退自如":i32}, error out=w768:errorcluster)
            n232 = Unbundle By Name(w773) -> ("进退自如"=w770:i32, "Row"=w769:i32)
            n233 = in-place {
              in-place-border: w770 -> [w783]
              in-place-border: w770 -> [w781]
              in-place-border: w769 -> [w777]
              n234 = in-place-cluster #5(w772) -> ("进表寄存器"=w782:string[][], "退表寄存器"=w780:string[][])  [unwired: 1 out]
              n235 = case shown="1, 默认" w781 {
                tunnel: w782 -> [w787 w793]
                tunnel: w780 -> [w788 w792]
                tunnel: [w788 w790] -> w779
                tunnel: [w785 w793] -> w778
                tunnel: w777 -> [w786 w791]
                frame 1, Default {
                  n236 = call "Add-data.vi"("F-UP/T-Down"=TRUE, "Indix"=w786, "数组"=w787) -> ("输出数组"=w785:string[][])  [unwired: 8 in]
                  n237 = property on="编辑显示进表" class="多列列表框 (严格)"("ItemNames"=w785) -> ()  [unwired: 2 in, 2 out]
                }
                frame 2 {
                  n238 = call "Add-data.vi"("F-UP/T-Down"=TRUE, "Indix"=w791, "数组"=w792) -> ("输出数组"=w790:string[][])  [unwired: 8 in]
                  n239 = property on="编辑显示退表" class="多列列表框 (严格)"("ItemNames"=w790) -> ()  [unwired: 2 in, 2 out]
                }
              }
              n240 = in-place-cluster #5("进退自如"=w783, "进表寄存器"=w778, "退表寄存器"=w779) -> (w771:T4)
            }
            n241 = call-poly <vilib>:"Delacor_lib_QMH_Enqueue Message (poly).vi"("error in"=w768, "Message"="Add-Edit-data", "Message Queue in"=w767) -> ("error out"=w766:errorcluster)  [unwired: 7 in, 1 out]
          }
          frame "Add-Edit-data" {
            n242 = Unbundle By Name(w807) -> ("Databas"=w802:refnum<class "Database_access.lvclass">, "选择表名"=w806:string, "进退自如"=w805:u8, "进表寄存器"=w797:string[][], "退表寄存器"=w796:string[][])
            n243 = call "Indicator-string.vi"("字符串"=w806) -> ("退表名"=w803:string, "进表名"=w804:string)  [unwired: 8 in, 1 out]
            n244 = case shown="1, 默认" w805 {
              tunnel: w804 -> [w819 _]
              tunnel: w803 -> [_ w821]
              tunnel: [w819 w821] -> w799
              tunnel: w797 -> [w818 _]
              tunnel: w796 -> [_ w820]
              tunnel: [w818 w820] -> w795
              frame 1, Default {
              }
              frame 2 {
              }
            }
            n245 = call-dynamic "Truncate_Table.vi"("Name"=w799, "Database_access 输入"=w802) -> ("error out"=w800:errorcluster, "Database_access 输出"=w801:refnum<class "Database_access.lvclass">)  [unwired: 8 in]
            n246 = for {
              tunnel: w795 -> [w810] mode=indexing
              tunnel: [w809] -> w794 mode=indexing
              n247 = Array To Cluster(array=w810) -> (cluster=w809:T20)
            }
            n248 = for {
              tunnel: w801 -> [w817]
              tunnel: [w816] -> _
              tunnel: w800 -> [w815]
              tunnel: [w814] -> _
              tunnel: w799 -> [w813]
              tunnel: string[] ["序号", "行为", "动作", "数值", "数据类型"] ("columns") -> [w812]
              tunnel: w794 -> [w811] mode=indexing
              n249 = call-dynamic "Insert_database.vi"("data"=w811, "error in (no error)"=w815, "columns"=w812, "table"=w813, "Database_access 输入"=w817) -> ("error out"=w814:errorcluster, "Database_access 输出"=w816:refnum<class "Database_access.lvclass">)  [unwired: 5 in]
            }
          }
          frame "Delete" {
            n250 = Variant To Data(error in=w833, type=cluster{"Row":i32, "进退自如":i32} {"Row"=0, "进退自如"=2}, Variant=w832) -> (data=w830:cluster{"Row":i32, "进退自如":i32}, error out=w825:errorcluster)
            n251 = Unbundle By Name(w830) -> ("进退自如"=w827:i32, "Row"=w826:i32)
            n252 = in-place {
              in-place-border: w827 -> [w840]
              in-place-border: w827 -> [w838]
              in-place-border: w826 -> [w834]
              n253 = in-place-cluster #6(w829) -> ("进表寄存器"=w839:string[][], "退表寄存器"=w837:string[][])  [unwired: 1 out]
              n254 = case shown="2" w838 {
                tunnel: w839 -> [w843 w848]
                tunnel: w837 -> [w844 w847]
                tunnel: [w844 w845] -> w836
                tunnel: [w841 w848] -> w835
                tunnel: w834 -> [w842 w846]
                frame 1, Default {
                  n255 = call "Delte-data.vi"("Indix"=w842, "数组"=w843) -> ("输出数组"=w841:string[][])  [unwired: 9 in]
                  n256 = property on="编辑显示进表" class="多列列表框 (严格)"("ItemNames"=w841) -> ()  [unwired: 2 in, 2 out]
                }
                frame 2 {
                  n257 = call "Delte-data.vi"("Indix"=w846, "数组"=w847) -> ("输出数组"=w845:string[][])  [unwired: 9 in]
                  n258 = property on="编辑显示退表" class="多列列表框 (严格)"("ItemNames"=w845) -> ()  [unwired: 2 in, 2 out]
                }
              }
              n259 = in-place-cluster #6("进退自如"=w840, "进表寄存器"=w835, "退表寄存器"=w836) -> (w828:T4)
            }
            n260 = call-poly <vilib>:"Delacor_lib_QMH_Enqueue Message (poly).vi"("error in"=w825, "Message"="Delete-Edit-data", "Message Queue in"=w823) -> ("error out"=w824:errorcluster)  [unwired: 7 in, 1 out]
          }
          frame "Delete-Edit-data" {
            n261 = Unbundle By Name(w862) -> ("Databas"=w857:refnum<class "Database_access.lvclass">, "选择表名"=w861:string, "进退自如"=w860:u8, "进表寄存器"=w852:string[][], "退表寄存器"=w851:string[][])
            n262 = call "Indicator-string.vi"("字符串"=w861) -> ("退表名"=w858:string, "进表名"=w859:string)  [unwired: 8 in, 1 out]
            n263 = case shown="2" w860 {
              tunnel: w859 -> [w874 _]
              tunnel: w858 -> [_ w876]
              tunnel: [w874 w876] -> w854
              tunnel: w852 -> [w873 _]
              tunnel: w851 -> [_ w875]
              tunnel: [w873 w875] -> w850
              frame 1, Default {
              }
              frame 2 {
              }
            }
            n264 = call-dynamic "Truncate_Table.vi"("Name"=w854, "Database_access 输入"=w857) -> ("error out"=w855:errorcluster, "Database_access 输出"=w856:refnum<class "Database_access.lvclass">)  [unwired: 8 in]
            n265 = for {
              tunnel: w850 -> [w865] mode=indexing
              tunnel: [w864] -> w849 mode=indexing
              n266 = Array To Cluster(array=w865) -> (cluster=w864:T20)
            }
            n267 = for {
              tunnel: w856 -> [w872]
              tunnel: [w871] -> _
              tunnel: w855 -> [w870]
              tunnel: [w869] -> _
              tunnel: w854 -> [w868]
              tunnel: string[] ["序号", "行为", "动作", "数值", "数据类型"] ("columns") -> [w867]
              tunnel: w849 -> [w866] mode=indexing
              n268 = call-dynamic "Insert_database.vi"("data"=w866, "error in (no error)"=w870, "columns"=w867, "table"=w868, "Database_access 输入"=w872) -> ("error out"=w869:errorcluster, "Database_access 输出"=w871:refnum<class "Database_access.lvclass">)  [unwired: 5 in]
            }
          }
          frame "-----------------D-----------------" {
          }
          frame "Choose_Edit" {
            # "拿出表名"
            n269 = Variant To Data(error in=w898, type=0 ("Row"), Variant=w899) -> (data=w897:i32, error out=w896:errorcluster)
            n270 = Unbundle By Name(w901) -> ("Databas"=w902:refnum<class "Database_access.lvclass">, "总览表寄存器"=w904:string[][])
            n271 = Index Array(array=w904, index (row) #1=w897, index (col) #1=1 ("禁用的索引 (列)")) -> (element #1=w880:string, element #2=w879:string)  [unwired: 2 in]
            n272 = call "Indicator-string.vi"("字符串"=w879) -> ("退表名"=w893:string, "进表名"=w884:string)  [unwired: 8 in, 1 out]
            n273 = call-dynamic "Read_database.vi"("table"=w884, "Database_access 输入"=w902) -> ("error out"=w892:errorcluster, "data"=w891:variant[][], "Database_access 输出"=w894:refnum<class "Database_access.lvclass">)  [unwired: 7 in]
            n274 = call "StringArr-type"("database variant"=w891) -> ("error out"=w886:errorcluster, "data"=w882:string[][])  [unwired: 9 in]
            n275 = call-dynamic "Read_database.vi"("error in (no error)"=w892, "table"=w893, "Database_access 输入"=w894) -> ("error out"=w885:errorcluster, "data"=w890:variant[][])  [unwired: 6 in, 1 out]
            n276 = property on="编辑显示进表" class="多列列表框 (严格)"(error in=w886, "ItemNames"=w882) -> (error out=w887:errorcluster)  [unwired: 1 in, 1 out]
            n277 = call "StringArr-type"("error in (no error)"=w887, "database variant"=w890) -> ("error out"=w888:errorcluster, "data"=w881:string[][])  [unwired: 8 in]
            n278 = property on="编辑显示退表" class="多列列表框 (严格)"(error in=w888, "ItemNames"=w881) -> (error out=w889:errorcluster)  [unwired: 1 in, 1 out]
            n279 = case shown="错误" w885 {
              tunnel: w880 -> [_ w905]
              frame No Error {
              }
              frame Error {
                n280 = Format Into String(format string="数据库无%S项\n请检查" ("字符串"), w905) -> (resulting string=w906:string)  [unwired: 2 in, 1 out]
                n281 = One Button Dialog(message=w906) -> ()  [unwired: 1 in, 1 out]
              }
            }
            n282 = Bundle By Name(cluster=w901, "进表寄存器"=w882, "退表寄存器"=w881, "选择表名"=w879) -> (w883:T4)
            n283 = Merge Errors(w889, w896) -> (w895:errorcluster)
          }
          frame "Edit-A" {
            n284 = Variant To Data(error in=w919, type=T10 {"单元格位置"={"Row"=0, "Column"=0}, "控件引用"=refnum, "进退自如"=0}, Variant=w918) -> (data=w915:T10, error out=w917:errorcluster)
            n285 = Unbundle By Name(w915) -> ("单元格位置.Row"=w910:i32, "单元格位置.Column"=w913:i32, "单元格位置"=w908:cluster{"Row":i32, "Column":i32}, "控件引用"=w912:refnum<vi>)
            n286 = Unbundle By Name(w914) -> ("总览表寄存器"=w911:string[][])
            n287 = Bundle By Name(cluster=w914, "行列号"=w908) -> (w909:T4)
            n288 = case shown="0, 默认" w913 {
              selector: w913 -> [_ w922]
              tunnel: w908 -> [_ w925]
              tunnel: w912 -> [_ w926]
              tunnel: w911 -> [_ w924]
              tunnel: w910 -> [_ w923]
              frame 0, Default {
              }
              frame 1 {
                n289 = property on="属性节点" class="MCListbox (严格)"(reference=w926, "ActiveCell"=w925) -> ("ActiveCellPos"=w921:T1)  [unwired: 1 in, 2 out]
                n290 = Index Array(array=w924, index (row)=w923, index (col)=w922) -> (element=w920:string)
                n291 = property on="Valued" class="Str"("Value"=w920, "Position"=w921) -> ()  [unwired: 2 in, 2 out]
              }
            }
          }
          frame "Modify-V" {
            n292 = Variant To Data(error in=w939, type="", Variant=w938) -> (data=w929:string, error out=w932:errorcluster)
            n293 = Unbundle By Name(w940) -> ("总览表寄存器"=w928:string[][], "行列号"=w936:cluster{"Row":i32, "Column":i32})
            n294 = call-poly <vilib>:"Delacor_lib_QMH_Enqueue Message (poly).vi"("error in"=w932, "Message Data"=w929, "Message"="Modify-data-V", "Message Queue in"=w931) -> ()  [unwired: 6 in, 2 out]
            n295 = Unbundle By Name(w936) -> ("Row"=w935:i32, "Column"=w934:i32)
            n296 = Replace Array Subset(array=w928, new element=w929, index (row)=w935, index (col)=w934) -> (w927:string[][])
            n297 = Bundle By Name(cluster=w940, "总览表寄存器"=w927) -> (w933:T4)
            n298 = property on="编辑显示总览" class="MCListbox (严格)"("ItemNames"=w927) -> ()  [unwired: 2 in, 2 out]
          }
          frame "Modify-data-V" {
            n299 = Variant To Data(error in=w943, type="", Variant=w948) -> (data=w947:string)  [unwired: 1 out]
            n300 = Unbundle By Name(w954) -> ("Databas"=w953:refnum<class "Database_access.lvclass">, "行列号.Row"=w945:i32)
            n301 = Increment(x=w945) -> (x+1=w950:i32)
            n302 = Format Into String(format string="WHERE 序号 = '%d'" ("格式字符串"), w950) -> (resulting string=w951:string)  [unwired: 2 in, 1 out]
            n303 = call-dynamic "Update_database.vi"("data"=w947, "condition"=w951, "columns"=string[] ["步骤名称"], "table"="总览", "Database_access 输入"=w953) -> ("error out"=w941:errorcluster)  [unwired: 5 in, 1 out]
            n304 = Merge Errors(w941, w943) -> (w942:errorcluster)
          }
          frame "Add_Table_Up" {
            n305 = Variant To Data(error in=w970, type=0 ("Row"), Variant=w971) -> (data=w966:i32, error out=w968:errorcluster)
            n306 = Unbundle By Name(w972) -> ("总览表寄存器"=w967:string[][])
            n307 = Two Button Dialog(message="痕迹将永远存在" ("消息"), 1:"后悔药" ("F按钮名称（“取消”）"), 2:"心意已决" ("T按钮名称（“确定”）")) -> (T button?=w964:bool)
            n308 = case shown="True" w964 {
              tunnel: w967 -> [w973 w980]
              tunnel: w966 -> [_ w979]
              tunnel: [w973 w975] -> w956
              tunnel: w960 -> [_ w978]
              tunnel: [_ w977] -> w958
              tunnel: [_ w974] -> w957
              frame False {
              }
              frame True {
                n309 = call "Add-table.vi"("Indix"=w979, "数组"=w980) -> ("New-table"=w974:string, "输出数组"=w975:string[][])  [unwired: 8 in]
                n310 = property on="编辑显示总览" class="MCListbox (严格)"("ItemNames"=w975) -> ()  [unwired: 2 in, 2 out]
                n311 = call-poly <vilib>:"Delacor_lib_QMH_Enqueue Message (poly).vi"("Message"="Add-Edit-Table", "Message Queue in"=w978) -> ("error out"=w977:errorcluster)  [unwired: 8 in, 1 out]
              }
            }
            n312 = Array Size(array=w956) -> (size(s)=w955:i32[])
            n313 = Merge Errors(w958, w968) -> (w959:errorcluster)
            n314 = Bundle By Name(cluster=w972, "总览表寄存器"=w956, "New-table"=w957, "总览大小"=w955) -> (w965:T4)
          }
          frame "Add_Table_Down" {
            n315 = Variant To Data(error in=w996, type=0 ("Row"), Variant=w997) -> (data=w992:i32, error out=w994:errorcluster)
            n316 = Unbundle By Name(w998) -> ("总览表寄存器"=w993:string[][])
            n317 = Two Button Dialog(message="痕迹将永远存在" ("消息"), 1:"后悔药" ("F按钮名称（“取消”）"), 2:"心意已决" ("T按钮名称（“确定”）")) -> (T button?=w990:bool)
            n318 = case shown="True" w990 {
              tunnel: w993 -> [w999 w1007]
              tunnel: w992 -> [_ w1006]
              tunnel: [w999 w1002] -> w982
              tunnel: w986 -> [_ w1005]
              tunnel: [_ w1004] -> w984
              tunnel: [_ w1001] -> w983
              frame False {
              }
              frame True {
                n319 = call "Add-table.vi"("F-UP/T-Down"=TRUE, "Indix"=w1006, "数组"=w1007) -> ("New-table"=w1001:string, "输出数组"=w1002:string[][])  [unwired: 7 in]
                n320 = property on="编辑显示总览" class="MCListbox (严格)"("ItemNames"=w1002) -> ()  [unwired: 2 in, 2 out]
                n321 = call-poly <vilib>:"Delacor_lib_QMH_Enqueue Message (poly).vi"("Message"="Add-Edit-Table", "Message Queue in"=w1005) -> ("error out"=w1004:errorcluster)  [unwired: 8 in, 1 out]
              }
            }
            n322 = Array Size(array=w982) -> (size(s)=w981:i32[])
            n323 = Merge Errors(w984, w994) -> (w985:errorcluster)
            n324 = Bundle By Name(cluster=w998, "总览表寄存器"=w982, "New-table"=w983, "总览大小"=w981) -> (w991:T4)
          }
          frame "Add-Edit-Table" {
            w1008 = string[] ["序号", "行为", "动作", "数值", "数据类型"] ("columns")
            w1011 = T21 {"字符串"="1", "字符串 2"="", "字符串 3"="", "字符串 4"="", "字符串 5"=""}
            w1022 = T22 [{"column name"="序号", "data type"=enum."String", "size"=255, "allow null?"=TRUE}, {"column name"="行为", "data type"=enum."String", "size"=255, "allow null?"=TRUE}, {"column name"="动作", "data type"=enum."String", "size"=255, "allow null?"=TRUE}, {"column name"="数值", "data type"=enum."String", "size"=255, "allow null?"=TRUE}, {"column name"="数据类型", "data type"=enum."String", "size"=255, "allow null?"=TRUE}] ("column information")
            w1031 = "总览" ("Name")
            n325 = Unbundle By Name(w1035) -> ("Databas"=w1034:refnum<class "Database_access.lvclass">, "总览表寄存器"=w1029:string[][], "New-table"=w1025:string)
            n326 = for {
              tunnel: w1029 -> [w1037] mode=indexing
              tunnel: [w1036] -> w1028 mode=indexing
              n327 = Array To Cluster(array=w1037) -> (cluster=w1036:T25)
            }
            n328 = call-poly <vilib>:"Delacor_lib_QMH_Enqueue Message (poly).vi"("error in"=w1019, "Message"="In A", "Message Queue in"=w1020) -> ("error out"=w1018:errorcluster)  [unwired: 7 in, 1 out]
            n329 = call-dynamic "Truncate_Table.vi"("error in (no error)"=w1019, "Name"=w1031, "Database_access 输入"=w1034) -> ("error out"=w1032:errorcluster, "Database_access 输出"=w1033:refnum<class "Database_access.lvclass">)  [unwired: 7 in]
            n330 = for {
              tunnel: w1033 -> [w1044]
              tunnel: w1032 -> [w1043]
              tunnel: w1031 -> [w1042]
              tunnel: string[] ["序号", "步骤名称", "表名"] ("columns") -> [w1041]
              tunnel: w1028 -> [w1040] mode=indexing
              tunnel: [w1039] -> w1027
              tunnel: [w1038] -> w1026
              n331 = call-dynamic "Insert_database.vi"("data"=w1040, "error in (no error)"=w1043, "columns"=w1041, "table"=w1042, "Database_access 输入"=w1044) -> ("error out"=w1038:errorcluster, "Database_access 输出"=w1039:refnum<class "Database_access.lvclass">)  [unwired: 5 in]
            }
            n332 = call "Indicator-string.vi"("字符串"=w1025) -> ("退表名"=w1009:string, "进表名"=w1010:string)  [unwired: 8 in, 1 out]
            n333 = call-dynamic "Createt_Table.vi"("error in (no error)"=w1026, "column information"=w1022, "table"=w1010, "Database_access 输入"=w1027) -> ("error out"=w1023:errorcluster, "Database_access 输出"=w1024:refnum<class "Database_access.lvclass">)  [unwired: 6 in]
            n334 = call-dynamic "Createt_Table.vi"("error in (no error)"=w1023, "column information"=w1022, "table"=w1009, "Database_access 输入"=w1024) -> ("error out"=w1013:errorcluster, "Database_access 输出"=w1016:refnum<class "Database_access.lvclass">)  [unwired: 6 in]
            n335 = call-dynamic "Insert_database.vi"("data"=w1011, "error in (no error)"=w1013, "columns"=w1008, "table"=w1010, "Database_access 输入"=w1016) -> ("error out"=w1014:errorcluster, "Database_access 输出"=w1015:refnum<class "Database_access.lvclass">)  [unwired: 5 in]
            n336 = call-dynamic "Insert_database.vi"("data"=w1011, "error in (no error)"=w1014, "columns"=w1008, "table"=w1009, "Database_access 输入"=w1015) -> ("error out"=w1012:errorcluster)  [unwired: 5 in, 1 out]
            n337 = Merge Errors(w1012, w1018) -> (w1021:errorcluster)
          }
          frame "Delete_Table" {
            n338 = Variant To Data(error in=w1060, type=0 ("Row"), Variant=w1061) -> (data=w1056:i32, error out=w1058:errorcluster)
            n339 = Unbundle By Name(w1062) -> ("总览表寄存器"=w1057:string[][])
            n340 = Two Button Dialog(message="失去的将永远失去" ("消息"), 1:"后悔药" ("F按钮名称（“取消”）"), 2:"心意已决" ("T按钮名称（“确定”）")) -> (T button?=w1054:bool)
            n341 = case shown="True" w1054 {
              tunnel: w1057 -> [w1063 w1070]
              tunnel: w1056 -> [_ w1069]
              tunnel: [w1063 w1065] -> w1046
              tunnel: w1050 -> [_ w1068]
              tunnel: [_ w1067] -> w1048
              tunnel: [_ w1064] -> w1047
              frame False {
              }
              frame True {
                n342 = call "Delte-table.vi"("Indix"=w1069, "数组"=w1070) -> ("Old-table"=w1064:string, "输出数组"=w1065:string[][])  [unwired: 8 in]
                n343 = property on="编辑显示总览" class="MCListbox (严格)"("ItemNames"=w1065) -> ()  [unwired: 2 in, 2 out]
                n344 = call-poly <vilib>:"Delacor_lib_QMH_Enqueue Message (poly).vi"("Message"="Delte-Edit-Table", "Message Queue in"=w1068) -> ("error out"=w1067:errorcluster)  [unwired: 8 in, 1 out]
              }
            }
            n345 = Array Size(array=w1046) -> (size(s)=w1045:i32[])
            n346 = Merge Errors(w1048, w1058) -> (w1049:errorcluster)
            n347 = Bundle By Name(cluster=w1062, "总览表寄存器"=w1046, "Old-table"=w1047, "总览大小"=w1045) -> (w1055:T4)
          }
          frame "Delte-Edit-Table" {
            w1087 = "总览" ("Name")
            n348 = Unbundle By Name(w1091) -> ("Databas"=w1090:refnum<class "Database_access.lvclass">, "总览表寄存器"=w1085:string[][], "Old-table"=w1081:string)
            n349 = for {
              tunnel: w1085 -> [w1093] mode=indexing
              tunnel: [w1092] -> w1084 mode=indexing
              n350 = Array To Cluster(array=w1093) -> (cluster=w1092:T25)
            }
            n351 = call-poly <vilib>:"Delacor_lib_QMH_Enqueue Message (poly).vi"("error in"=w1073, "Message"="In A", "Message Queue in"=w1074) -> ("error out"=w1072:errorcluster)  [unwired: 7 in, 1 out]
            n352 = call-dynamic "Truncate_Table.vi"("error in (no error)"=w1073, "Name"=w1087, "Database_access 输入"=w1090) -> ("error out"=w1088:errorcluster, "Database_access 输出"=w1089:refnum<class "Database_access.lvclass">)  [unwired: 7 in]
            n353 = for {
              tunnel: w1089 -> [w1100]
              tunnel: w1088 -> [w1099]
              tunnel: w1087 -> [w1098]
              tunnel: string[] ["序号", "步骤名称", "表名"] ("columns") -> [w1097]
              tunnel: w1084 -> [w1096] mode=indexing
              tunnel: [w1095] -> w1083
              tunnel: [w1094] -> w1082
              n354 = call-dynamic "Insert_database.vi"("data"=w1096, "error in (no error)"=w1099, "columns"=w1097, "table"=w1098, "Database_access 输入"=w1100) -> ("error out"=w1094:errorcluster, "Database_access 输出"=w1095:refnum<class "Database_access.lvclass">)  [unwired: 5 in]
            }
            n355 = call "Indicator-string.vi"("字符串"=w1081) -> ("退表名"=w1077:string, "进表名"=w1080:string)  [unwired: 8 in, 1 out]
            n356 = call-dynamic "Delete_Table.vi"("error in (no error)"=w1082, "table"=w1080, "Database_access 输入"=w1083) -> ("error out"=w1078:errorcluster, "Database_access 输出"=w1079:refnum<class "Database_access.lvclass">)  [unwired: 7 in]
            n357 = call-dynamic "Delete_Table.vi"("error in (no error)"=w1078, "table"=w1077, "Database_access 输入"=w1079) -> ("error out"=w1075:errorcluster)  [unwired: 7 in, 1 out]
            n358 = Merge Errors(w1075, w1072) -> (w1076:errorcluster)
          }
          frame "In A" {
            n359 = Unbundle By Name(w1104) -> ("总览大小"=w1103:i32[])
            n360 = Index Array(array=w1103) -> (element=w1107:i32)  [unwired: 1 in]
            n361 = Initialize Array(37, w1107) -> (w1101:i32[])
            n362 = property on="任务显示" class="MCListbox (严格)"("ItemSyms"=w1101) -> (error out=w1105:errorcluster)  [unwired: 2 in, 1 out]
            n363 = Merge Errors(w1105, w1109) -> (w1106:errorcluster)
            n364 = Bundle By Name(cluster=w1104, "项符号"=w1101) -> (w1102:T4)
          }
          frame "-----------------E-----------------" {
          }
          frame "Modify" {
            n365 = Variant To Data(error in=w1127, type="", Variant=w1126) -> (data=w1112:string, error out=w1115:errorcluster)
            n366 = Unbundle By Name(w1128) -> ("进退自如"=w1117:bool, "进表寄存器"=w1125:string[][], "退表寄存器"=w1124:string[][], "行列号"=w1121:cluster{"Row":i32, "Column":i32})
            n367 = call-poly <vilib>:"Delacor_lib_QMH_Enqueue Message (poly).vi"("error in"=w1115, "Message Data"=w1112, "Message"="Modify-data", "Message Queue in"=w1114) -> ()  [unwired: 6 in, 2 out]
            n368 = Select(t=w1125, s=w1117, f=w1124) -> (s? t:f=w1123:string[][])
            n369 = Unbundle By Name(w1121) -> ("Row"=w1120:i32, "Column"=w1119:i32)
            n370 = Replace Array Subset(array=w1123, new element=w1112, index (row)=w1120, index (col)=w1119) -> (w1116:string[][])
            n371 = case shown="False" w1117 {
              tunnel: w1128 -> [w1131 w1134]
              tunnel: [w1130 w1133] -> w1118
              tunnel: w1116 -> [w1129 w1132]
              frame True {
                n372 = Bundle By Name(cluster=w1131, "进表寄存器"=w1129) -> (w1130:T4)
                n373 = property on="编辑显示进表" class="MCListbox (严格)"("ItemNames"=w1129) -> ()  [unwired: 2 in, 2 out]
              }
              frame False {
                n374 = Bundle By Name(cluster=w1134, "退表寄存器"=w1132) -> (w1133:T4)
                n375 = property on="编辑显示退表" class="MCListbox (严格)"("ItemNames"=w1132) -> ()  [unwired: 2 in, 2 out]
              }
            }
          }
          frame "Modify-data" {
            n376 = Variant To Data(error in=w1136, type="", Variant=w1142) -> (data=w1141:string)  [unwired: 1 out]
            n377 = Unbundle By Name(w1154) -> ("Databas"=w1149:refnum<class "Database_access.lvclass">, "进退自如"=w1150:bool, "选择表名"=w1153:string, "行列号.Row"=w1144:i32, "行列号.Column"=w1139:i32)
            n378 = Increment(x=w1144) -> (x+1=w1145:i32)
            n379 = call "Indicator-string.vi"("字符串"=w1153) -> ("退表名"=w1152:string, "进表名"=w1151:string)  [unwired: 8 in, 1 out]
            n380 = Select(t=w1151, s=w1150, f=w1152) -> (s? t:f=w1148:string)
            n381 = Format Into String(format string="WHERE 序号 = '%d'" ("格式字符串"), w1145) -> (resulting string=w1146:string)  [unwired: 2 in, 1 out]
            n382 = Index Array(array=string[] ["序号", "行为", "动作", "数值", "数据类型"] ("columns"), index=w1139) -> (element=w1138:string)
            n383 = Build Array(w1138) -> (w1137:string[])
            n384 = call-dynamic "Update_database.vi"("data"=w1141, "condition"=w1146, "error in (no error)"=w1136, "columns"=w1137, "table"=w1148, "Database_access 输入"=w1149) -> ("error out"=w1135:errorcluster)  [unwired: 4 in, 1 out]
          }
          frame "-----------------F-----------------" {
          }
          frame "Parse task" {
            # "使用移位寄存器能让内存少复制一次"
            # "不能直接用，防止中间态导致数据变化\n好像没有中间态存在"
            # "拿到所有需要的做的表名"
            n385 = Unbundle By Name(w1167) -> ("总览表寄存器"=w1166:string[][], "项符号"=w1164:i32[])
            n386 = Index Array(array=w1166, index (col)=2 ("禁用的索引 (列)")) -> (element=w1163:string[])  [unwired: 1 in]
            n387 = for {
              tunnel: w1164 -> [w1171] mode=indexing
              tunnel: w1163 -> [w1169] mode=indexing
              tunnel: [w1169] -> w1157 mode=indexing if=w1168
              n388 = Equal?(x=w1171, y=38) -> (x = y?=w1168:bool)
            }
            n389 = call-poly <vilib>:"Delacor_lib_QMH_Enqueue Message (poly).vi"("error in"=w1161, "Message"="Take task", "Message Queue in"=w1160) -> ("error out"=w1159:errorcluster)  [unwired: 7 in, 1 out]
            n390 = Bundle By Name(cluster=w1167, "Choosed task"=w1157) -> (w1162:T4)
          }
          frame "Take task" {
            n391 = Unbundle By Name(w1173) -> ("Choosed task"=w1172:string[])
            n392 = Empty Array?(array=w1172) -> (empty?=w1177:bool)
            n393 = case shown="False" w1177 {
              tunnel: w1176 -> [w1181 w1183]
              tunnel: [w1182 w1183] -> w1175
              tunnel: w1174 -> [w1179 _]
              frame False {
                n394 = property on="开始" class="button3 (严格)"("DisabledEnum"=T16."Disabled and Grayed Out" ("禁用")) -> ()  [unwired: 2 in, 2 out]
                n395 = call-poly <vilib>:"Delacor_lib_QMH_Enqueue Message (poly).vi"("error in"=w1181, "Message"="Start 1", "Message Queue in"=w1179) -> ("error out"=w1182:errorcluster)  [unwired: 7 in, 1 out]
              }
              frame True {
              }
            }
          }
          frame "End" {
            n396 = property on="开始" class="button3 (严格)"("DisabledEnum"=T16."Enabled" ("禁用")) -> ()  [unwired: 2 in, 2 out]
          }
          frame "-----------------G-----------------" {
          }
          frame "Start 1" {
            # "每次只取一个表，读取表单不会很慢，减少运存开支\n从业务上来说，一个表存储了一个试验步骤，这个步骤结束了，在下个步骤之间，这个间隔是无所谓的"
            n397 = Unbundle By Name(w1201) -> ("Choosed task"=w1200:string[], "Databas"=w1198:refnum<class "Database_access.lvclass">)
            n398 = call-poly <vilib>:"Delacor_lib_QMH_Enqueue Message (poly).vi"("error in"=w1193, "Message"="Send", "Message Queue in"=w1192) -> ()  [unwired: 7 in, 2 out]
            n399 = call "Add Flag.vi"("数组IN"=w1200) -> ("数组"=w1202:string[], "table1"=w1199:string)  [unwired: 9 in]
            n400 = call-dynamic "Read_database.vi"("error in (no error)"=w1193, "table"=w1199, "Database_access 输入"=w1198) -> ("error out"=w1196:errorcluster, "data"=w1197:variant[][])  [unwired: 6 in, 1 out]
            n401 = call "StringArr-type"("error in (no error)"=w1196, "database variant"=w1197) -> ("error out"=w1191:errorcluster, "data"=w1195:string[][])  [unwired: 8 in]
            n402 = call "Add-size.vi"("数组"=w1195) -> ("添加的数组"=w1189:string[][])  [unwired: 10 in]
            n403 = Bundle By Name(cluster=w1201, "Remaining table"=w1202, "Remaining Process"=w1195, "Execute Process"=w1189) -> (w1203:T4)
            n404 = call "Refursh-UI.vi"("error in"=w1191, "ARR"=w1189) -> ("error out"=w1190:errorcluster)  [unwired: 9 in]
          }
          frame "Start 2" {
            n405 = Unbundle By Name(w1218) -> ("Remaining table"=w1210:string[], "Databas"=w1217:refnum<class "Database_access.lvclass">)
            n406 = call-poly <vilib>:"Delacor_lib_QMH_Enqueue Message (poly).vi"("error in"=w1212, "Message"="Send", "Message Queue in"=w1211) -> ()  [unwired: 7 in, 2 out]
            n407 = Delete From Array(array=w1210, index=0 ("索引")) -> (deleted portion=w1208:string, array with subset deleted=w1207:string[])  [unwired: 1 in]
            n408 = call-dynamic "Read_database.vi"("error in (no error)"=w1212, "table"=w1208, "Database_access 输入"=w1217) -> ("error out"=w1215:errorcluster, "data"=w1216:variant[][])  [unwired: 6 in, 1 out]
            n409 = call "StringArr-type"("error in (no error)"=w1215, "database variant"=w1216) -> ("error out"=w1205:errorcluster, "data"=w1206:string[][])  [unwired: 8 in]
            n410 = call "Add-size.vi"("数组"=w1206) -> ("添加的数组"=w1214:string[][])  [unwired: 10 in]
            n411 = call "Refursh-UI.vi"("error in"=w1205, "ARR"=w1206) -> ("error out"=w1204:errorcluster)  [unwired: 9 in]
            n412 = Bundle By Name(cluster=w1218, "Remaining table"=w1207, "Remaining Process"=w1206, "Execute Process"=w1214) -> (w1219:T4)
          }
          frame "Send" {
            n413 = in-place {
              in-place-border: [w1225] -> w1222
              n414 = in-place-cluster #7(w1224) -> ("Remaining Process"=w1230:string[][])
              n415 = Delete From Array(array=w1230, length=1 ("长度"), index (row)=0 ("索引 (行)")) -> (deleted portion=w1226:string[][], array with subset deleted=w1229:string[][])  [unwired: 1 in]
              n416 = Index Array(array=w1226) -> (element=w1225:string[])  [unwired: 2 in]
              n417 = in-place-cluster #7("Remaining Process"=w1229) -> (w1223:T4)
            }
            n418 = call "Send task.vi"("error in"=w1221, "Task"=w1222) -> ("error out"=w1220:errorcluster)  [unwired: 9 in]
          }
          frame "Receive end" {
            # "做完一步返回一个指令"
            n419 = Variant To Data(error in=w1246, type=T14 {"Arr"=[]} ("Receive end Argument"), Variant=w1245) -> (data=w1243:T14, error out=w1238:errorcluster)
            n420 = Unbundle By Name(w1243) -> ("Arr"=w1235:string[])
            n421 = Index Array(array=w1235) -> (element=w1242:string)  [unwired: 1 in]
            n422 = Decimal String To Number(string=w1242) -> (number=w1239:i32)  [unwired: 2 in, 1 out]
            n423 = Decrement(x=w1239) -> (x-1=w1233:i32)
            n424 = in-place {
              in-place-border: w1233 -> [w1250]
              in-place-border: w1235 -> [w1249]
              in-place-border: [w1247] -> w1231
              n425 = in-place-cluster #8(w1241) -> ("Execute Process"=w1251:string[][])
              n426 = Replace Array Subset(array=w1251, new element=w1249, index (row)=w1250) -> (w1248:string[][])  [unwired: 1 in]
              n427 = in-place-cluster #8("Execute Process"=w1248) -> (w1240:T4)
              n428 = call "Refursh-UI.vi"("ARR"=w1248) -> ("error out"=w1247:errorcluster)  [unwired: 10 in]
            }
            n429 = call-poly <vilib>:"Delacor_lib_QMH_Enqueue Message (poly).vi"("error in"=w1238, "Message"="Judge NextStep", "Message Queue in"=w1237) -> ("error out"=w1236:errorcluster)  [unwired: 7 in, 1 out]
            n430 = Merge Errors(w1231, w1236) -> (w1232:errorcluster)
          }
          frame "Judge NextStep" {
            n431 = in-place {
              in-place-border: [w1266] -> w1258
              n432 = in-place-cluster #9(w1260) -> ("Remaining Process"=w1269:string[][], "Remaining table"=w1267:string[])
              n433 = Empty Array?(array=w1267) -> (empty?=w1268:bool)
              n434 = Empty Array?(array=w1269) -> (empty?=w1270:bool)
              n435 = call "Bollen-numb.vi"("布尔 2"=w1268, "布尔"=w1270) -> ("数字"=w1266:u32)  [unwired: 9 in]
              n436 = in-place-cluster #9("Remaining Process"=w1269, "Remaining table"=w1267) -> (w1259:T4)
            }
            n437 = case shown="3" w1258 {
              tunnel: ["Send" ("Message") "Start 2" ("Message") "End" ("Message")] -> w1253
              frame 2, 6, Default {
              }
              frame 3 {
              }
              frame 7 {
              }
            }
            n438 = case shown="True" "暂停" {
              tunnel: w1253 -> [w1264 _]
              tunnel: [w1264 "Pause" ("Message")] -> w1252
              frame False {
              }
              frame True {
              }
            }
            n439 = call-poly <vilib>:"Delacor_lib_QMH_Enqueue Message (poly).vi"("error in"=w1256, "Message Data"=w1253, "Message"=w1252, "Message Queue in"=w1257) -> ("error out"=w1254:errorcluster)  [unwired: 6 in, 1 out]
          }
          frame "Pause" {
            # "合理的清除"
            n440 = Variant To Data(error in=w1285, type="" ("暂停指令"), Variant=w1284) -> (data=w1281:string, error out=w1280:errorcluster)
            n441 = in-place {
              in-place-border: w1281 -> [w1292]
              in-place-border: [w1291] -> w1274
              n442 = in-place-cluster #10(w1283) -> ("暂停指令"=w1291:string)
              n443 = in-place-cluster #10("暂停指令"=w1292) -> (w1277:T4)
            }
            n444 = call <vilib>:"Clear Errors.vi"("error in (no error)"=w1280, "specific error code to clear (0: all)"=91) -> ("error out"=w1276:errorcluster)  [unwired: 4 in, 1 out]
            n445 = local read "暂停"() -> (w1272:bool)
            n446 = Empty String/Path?(string/path=w1274) -> (empty?=w1273:bool)
            n447 = Or(x=w1273, y=w1272) -> (x .or. y?=w1271:bool)
            n448 = case shown="False" w1271 {
              tunnel: w1276 -> [w1289 w1290]
              tunnel: w1279 -> [w1288 _]
              tunnel: [w1287 w1290] -> w1278
              tunnel: w1274 -> [w1286 _]
              frame False {
                n449 = call-poly <vilib>:"Delacor_lib_QMH_Enqueue Message (poly).vi"("error in"=w1289, "Message"=w1286, "Message Queue in"=w1288) -> ("error out"=w1287:errorcluster)  [unwired: 7 in, 1 out]
              }
              frame True {
              }
            }
          }
          frame "Stop" {
            # "当正在执行的命令返回之后，在去执行"
            # "只留当前正在执行的退出表单，并且立即执行"
            n450 = in-place {
              n451 = in-place-cluster #11(w1298) -> ("Remaining table"=w1304:string[], "Status"=w1300:string)  [unwired: 1 out]
              n452 = call "n_2"("数组"=w1304) -> ("已删除的部分"=w1303:string[])  [unwired: 10 in]
              n453 = Concatenate Strings(w1300, "\n执行退出工序……" ("字符串")) -> (w1299:string)
              n454 = in-place-cluster #11("Remaining table"=w1303, "Remaining Process"=string[][] [], "Status"=w1299) -> (w1294:T4)
            }
            n455 = call-poly <vilib>:"Delacor_lib_QMH_Enqueue Message (poly).vi"("error in"=w1296, "Message"="Judge NextStep", "Message Queue in"=w1293) -> ("error out"=w1295:errorcluster)  [unwired: 7 in, 1 out]
          }
          frame "-----------------H-----------------" {
          }
          frame "逗你玩" {
          }
          frame "---Exit and Error Handling---" {
            # "Separator - The following cases handle errors and exit messages."
          }
          frame "Simulate MHL Error" {
            # "#DQMH_HowTo The 'Simulate MHL Error' button  illustrates how the MHL handles errors. This event is instructional in nature and can be removed."
            # "Simulate an error occurring at the MHL"
            n456 = call "Module Name--constant.vi"() -> ("Module Name"=w1312:string)  [unwired: 11 in]
            n457 = Format Into String(format string="Simulated error originating at Message Handling Loop in %s", w1312) -> (resulting string=w1313:string)  [unwired: 2 in, 1 out]
            n458 = call <vilib>:"Error Cluster From Error Code.vi"("show call chain? (False)"=TRUE, "error message (\"\")"=w1313, "error code (0)"=5001) -> ("error out"=w1317:errorcluster)  [unwired: 6 in]
            n459 = Merge Errors(w1319, w1317) -> (w1318:errorcluster)
          }
          frame "Error" {
            # "#DQMH_CodeRecommended - If the module is running in standalone mode (External Launch = FALSE), this code will pop up an error dialog and call the 'Exit' message if an error occurs. Add more fine-grained error management here."
            # "Error - Check the error message data and respond accordingly. This message is sent by the \"Error Handler\" VIs at the end of each loop in this application."
            n460 = property on="Property Node" class="Module Admin"(reference=w1322) -> ("Accessors:External Launch"=w1321:bool)  [unwired: 1 in, 2 out]
            n461 = Variant To Data(error in=w1330, type=errorcluster {"status"=FALSE, "code"=0, "source"=""} ("error constant"), Variant=w1324) -> (data=w1320:errorcluster, error out=w1328:errorcluster)
            n462 = local write "error out"(w1320) -> ()
            n463 = call "Error Reported.vi"("Error"=w1320) -> ()  [unwired: 10 in, 1 out]
            n464 = case shown="False" w1321 {
              tunnel: [w1335 _] -> w1327
              tunnel: w1323 -> [w1333 _]
              tunnel: w1320 -> [w1334 _]
              frame False {
                n465 = disable-structure shown="Default" {
                  disable-tunnel: w1334 -> [w1336 _]
                  frame condition #0 (active) {
                    # "If the module is running standalone, then pop up an error dialog and call the \"Exit\" message."
                    n466 = call <vilib>:"Simple Error Handler.vi"("error in (no error)"=w1336) -> ()  [unwired: 4 in, 5 out]
                  }
                  frame condition #1 {
                    # "To prevent the Simple Error Handler VI from being loaded (e.g. when deploying to a Real-Time target), add the Conditional Disable Symbol \"DQMH_Disable_SEH\" to your project and set it to TRUE."
                  }
                }
                n467 = call-poly <vilib>:"Delacor_lib_QMH_Enqueue Message (poly).vi"("Priority Message? (F)"=TRUE, "Message"="Exit", "Message Queue in"=w1333) -> ("error out"=w1335:errorcluster)  [unwired: 7 in, 1 out]
              }
              frame True {
                # "If the module was launched externally, calling the Error Reported broadcast VI is the only action performed by the \"Error\" message. The module's caller can then process the error appropriately."
              }
            }
            n468 = Merge Errors(w1328, w1327) -> (w1326:errorcluster)
          }
          frame "Exit" {
            w1345 = 91  # 91: not all Exit messages will have an argument
            w1347 = TRUE  # Stop the VI
            # "Release the message queue reference"
            # "#DQMH_CodeNeeded - Add any required cleanup code here."
            # "Exit - Exit the application."
            n469 = Variant To Data(error in=w1354, type=T9 {"Origin"="", "Exit via Stop Module Req?"=FALSE, "Wait for Module to stop?"=FALSE} ("Stop Argument"), Variant=w1346) -> (data=w1343:T9, error out=w1351:errorcluster)
            n470 = call <vilib>:"Clear Errors.vi"("error in (no error)"=w1351, "specific error code to clear (0: all)"=w1345) -> ("error out"=w1353:errorcluster)  [unwired: 4 in, 1 out]
            n471 = control-ref of="This VI"() -> (w1342:refnum<vi>)
            n472 = call-dynamic "Delacor_lib_QMH_Release Message Queue.vi"("error in"=w1353, "Message Queue"=w1348) -> ("error out"=w1352:errorcluster)  [unwired: 9 in]
            n473 = call "Handle Exit.vi"("Stop Argument"=w1343, "Admin in"=w1341, "VI reference"=w1342) -> ("error out"=w1350:errorcluster)  [unwired: 7 in, 1 out]
            n474 = Merge Errors(w1352, w1350) -> (w1349:errorcluster)
            n475 = Unbundle By Name(w1340) -> ("Databas"=w1339:refnum<class "Database_access.lvclass">)
            n476 = call "Error Reported.vi"("Error"=w1349) -> ()  [unwired: 10 in, 1 out]
            n477 = call-dynamic "Close-database.vi"("Database_access 输入"=w1339) -> ("error out"=w1337:errorcluster)  [unwired: 9 in, 1 out]
            n478 = Merge Errors(w1337, w1349) -> (w1338:errorcluster)
          }
          frame Default {
            # "'Default' case only runs if there is a message that isn't defined in any of the other cases.  Output a programming error."
            n479 = call "Module Name--constant.vi"() -> ("Module Name"=w1359:string)  [unwired: 11 in]
            n480 = Format Into String(format string="The invalid message string \"%s\" was received in the Message Handling Loop for module \"%s\".", w1360, w1359) -> (resulting string=w1355:string)  [unwired: 2 in, 1 out]
            n481 = call <vilib>:"Error Cluster From Error Code.vi"("show call chain? (False)"=TRUE, "error message (\"\")"=w1355, "error code (0)"=1) -> ("error out"=w1362:errorcluster)  [unwired: 6 in]
            n482 = Merge Errors(w1363, w1362) -> (w1364:errorcluster)
          }
        }
        n483 = Unbundle By Name(w300) -> ("Status"=→"logging":string)
        n484 = call-dynamic "Delacor_lib_QMH_Error Handler - Message Handling Loop.vi"("error in"=w303, "Message Queue in"=w302) -> ("dup error in"=w304:errorcluster)  [unwired: 8 in, 1 out]
      }
      n485 = while "DQMH_HELPER_LOOP" {
        shift-right: [w46] -> _
        shift-left: -1 -> [w45]
        shift-right: [w43] -> w29
        shift-left: w28 -> [w44]
        tunnel: w32 -> [w40]
        stop <- w42 stop-if-true
        w39 = "refursh helper"  # DQMH_HELPER_LOOP_NAME
        # "refursh helper"
        n486 = event "DQMH_HELPER_EVENT_STRUCTURE" shown="[2] <Auto-Process Request Events.Refursh-UI>: 用户事件" {
          selector: w44 -> [_ _ _]
          dyn-events: [_ _ _] -> w43
          timeout: w45 -> [_ _ _]
          tunnel: w45 -> [w47 w50 w53]
          tunnel: [w47 w50 w53] -> w46
          tunnel: [_ TRUE _] -> w42
          tunnel: [_ errorcluster {"status"=FALSE, "code"=0, "source"=""} ("error constant") w51] -> w41
          tunnel: w40 -> [_ _ _]
          event Timeout {
            n487 = event-data() -> ()  [unwired: 1 in, 1 out]
          }
          event User Event {
            n488 = event-data() -> ()  [unwired: 1 in, 1 out]
          }
          event User Event {
            # "Another Module called the \"Refursh-UI\" API Method."
            n489 = event-data() -> ("ARR"=w52:string[][])  [unwired: 1 in]
            n490 = property on="执行显示" class="MCListbox (严格)"("ItemNames"=w52) -> (error out=w51:errorcluster)  [unwired: 2 in, 1 out]
          }
        }
        n491 = call-dynamic "Delacor_lib_QMH_Error Handler - Helper Loop.vi"("Error Debug"=w39, "error in"=w41, "Message Queue in"=w40) -> ()  [unwired: 7 in, 2 out]
      }
      n492 = while {
        tunnel: w32 -> [w55]
        shift-right: [w58] -> w35
        shift-left: w33 -> [w59]
        tunnel: [w60] -> w37
        tunnel: w31 -> [w56]
        stop <- w57 stop-if-true
        # "Event Handling Loop"
        n493 = event "DQMH_EVENT_MAIN" shown="[32] <Auto-Process Request Events.Receive end>: 用户事件" {
          selector: w59 -> [_ _ _ _ _ _ _ _ _ _ _ _ _ _ _ _ _ _ _ _ _ _ _ _ _ _ _ _ _ _ _ _ _]
          dyn-events: [_ _ _ _ _ _ _ _ _ _ _ _ _ _ _ _ _ _ _ _ _ _ _ _ _ _ _ _ _ _ _ _ _] -> w58
          timeout: 500 -> [_ _ _ _ _ _ _ _ _ _ _ _ _ _ _ _ _ _ _ _ _ _ _ _ _ _ _ _ _ _ _ _ _]
          tunnel: [_ _ _ _ _ _ _ _ _ _ _ TRUE ("Discard?") _ _ _ _ _ _ _ _ _ _ _ _ _ _ _ _ _ _ _ _ _] -> w57
          tunnel: w55 -> [w66 w72 w79 w86 w89 _ w104 _ _ _ _ w128 _ w136 w148 w153 w170 w175 w191 w201 w218 w221 w238 w243 w248 _ w256 w259 w269 w277 w279 w290 w296]
          tunnel: [w67 w73 w80 w87 w96 w102 w105 _ _ w111 _ w131 _ w138 w147 w151 w168 w173 w189 w200 w216 _ w232 _ _ _ w255 w258 w270 w272 w280 w284 w291] -> w61
          tunnel: w56 -> [_ _ _ _ _ _ _ _ _ _ _ _ _ w135 _ _ _ _ _ _ _ _ _ _ _ _ _ _ _ _ _ _ _]
          event "Do Something <Replace Me>": Value Change {
            # "#DQMH_HowTo The 'Do Something' messages are instructional in nature and can be removed with the Tools > DQMH Consortium > DQMH > Event > Remove DQMH Event utility."
            # "This case is to test the \"Do Something\" Message when this VI runs stand alone"
            n494 = event-data() -> ()  [unwired: 1 in, 1 out]
            n495 = Bundle(cluster=T5 {"Do Something Msg"=""} ("Do Something Argument"), "Do Something Msg"="\"Do Something\" button pressed" ("\"Do Something\" button pressed")) -> (w62:T5)
            n496 = call-poly <vilib>:"Delacor_lib_QMH_Enqueue Message (poly).vi"("Message Data"=w62, "Message"="Do Something", "Message Queue in"=w66) -> ("error out"=w67:errorcluster)  [unwired: 7 in, 1 out]
          }
          event User Event {
            # "#DQMH_HowTo The 'Do Something' messages are instructional in nature and can be removed with the Tools > DQMH Consortium > DQMH > Event > Remove DQMH Event utility."
            # "Another Module called the \"Do Something\" API Method."
            n497 = event-data() -> ("Do Something Msg"=w69:string)  [unwired: 1 in]
            n498 = Bundle(cluster=T5 {"Do Something Msg"=""} ("Do Something Argument"), "Do Something Msg"=w69) -> (w68:T5)
            n499 = call-poly <vilib>:"Delacor_lib_QMH_Enqueue Message (poly).vi"("Message Data"=w68, "Message"="Do Something", "Message Queue in"=w72) -> ("error out"=w73:errorcluster)  [unwired: 7 in, 1 out]
          }
          event "Do Something Else <Replace Me>": Value Change {
            # "#DQMH_HowTo The 'Do Something' messages are instructional in nature and can be removed with the Tools > DQMH Consortium > DQMH > Event > Remove DQMH Event utility."
            # "This case is to test the \"Do Something Else\" Message when this VI runs stand alone"
            n500 = event-data() -> ()  [unwired: 1 in, 1 out]
            n501 = Bundle(cluster=T6 {"Do Something Else Msg"="", "X"=0.0} ("Do Something Else Argument"), "Do Something Else Msg"="\"Do Something Else\" button pressed: " ("\"Do Something Else\" button pressed"), "X"=42.0) -> (w76:T6)
            n502 = call-poly <vilib>:"Delacor_lib_QMH_Enqueue Message (poly).vi"("Message Data"=w76, "Message"="Do Something Else", "Message Queue in"=w79) -> ("error out"=w80:errorcluster)  [unwired: 7 in, 1 out]
          }
          event User Event {
            # "#DQMH_HowTo The 'Do Something' messages are instructional in nature and can be removed with the Tools > DQMH Consortium > DQMH > Event Remove DQMH Event utility."
            # "Another Module called the \"Do Something Else\" API Method."
            n503 = event-data() -> ("Do Something Else Msg"=w82:string, "X"=w81:dbl)  [unwired: 1 in]
            n504 = Bundle(cluster=T6 {"Do Something Else Msg"="", "X"=0.0} ("Do Something Else Argument"), "Do Something Else Msg"=w82, "X"=w81) -> (w83:T6)
            n505 = call-poly <vilib>:"Delacor_lib_QMH_Enqueue Message (poly).vi"("Message Data"=w83, "Message"="Do Something Else", "Message Queue in"=w86) -> ("error out"=w87:errorcluster)  [unwired: 7 in, 1 out]
          }
          event User Event {
            # "#DQMH_HowTo The 'Do Something' messages are instructional in nature and can be removed with the Tools > DQMH Consortium > DQMH > Event > Remove DQMH Event utility."
            # "Another Module called the \"Do Something Else and Wait for Reply\" API Method."
            n506 = event-data() -> ("Do Something Else Msg"=w92:string, "X"=w91:dbl, "Wait Notifier"=w90:refnum<notifier>, "wait for reply"=w88:bool)  [unwired: 1 in]
            n507 = Bundle(cluster=T7 {"Do Something Else Msg"="", "X"=0.0, "Wait Notifier"=refnum, "wait for reply"=FALSE} ("Do Something Else and Wait for Reply Argument"), "Do Something Else Msg"=w92, "X"=w91, "Wait Notifier"=w90, "wait for reply"=w88) -> (w93:T7)
            n508 = call-poly <vilib>:"Delacor_lib_QMH_Enqueue Message (poly).vi"("Message Data"=w93, "Message"="Do Something Else and Wait for Reply", "Message Queue in"=w89) -> ("error out"=w96:errorcluster)  [unwired: 7 in, 1 out]
          }
          event "Simulate EHL Error": Value Change {
            # "#DQMH_HowTo The 'Simulate EHL Error' button  illustrates how the EHL handles errors. This event is instructional in nature and can be removed."
            # "This case simulates an error being generated by the EHL"
            n509 = event-data() -> ()  [unwired: 1 in, 1 out]
            n510 = call "Module Name--constant.vi"() -> ("Module Name"=w99:string)  [unwired: 11 in]
            n511 = Format Into String(format string="Simulated error originating at Event Handling Loop in %s", w99) -> (resulting string=w100:string)  [unwired: 2 in, 1 out]
            n512 = call <vilib>:"Error Cluster From Error Code.vi"("show call chain? (False)"=TRUE, "error message (\"\")"=w100, "error code (0)"=5000) -> ("error out"=w102:errorcluster)  [unwired: 6 in]
          }
          event "Simulate MHL Error": Value Change {
            # "#DQMH_HowTo The 'Simulate MHL Error' button  illustrates how the MHL handles errors. This event is instructional in nature and can be removed."
            # "This case simulates an error being generated by the MHL"
            n513 = event-data() -> ()  [unwired: 1 in, 1 out]
            n514 = call-poly <vilib>:"Delacor_lib_QMH_Enqueue Message (poly).vi"("Message"="Simulate MHL Error", "Message Queue in"=w104) -> ("error out"=w105:errorcluster)  [unwired: 8 in, 1 out]
          }
          event User Event {
            # "Show the panel of this VI, and send a status updated message to let listeners know."
            # "Another Module called the \"Show Panel\" API Method."
            n515 = event-data() -> ()  [unwired: 1 in, 1 out]
            n516 = control-ref of="This VI"() -> (w107:refnum<vi>)
            n517 = call "Open VI Panel.vi"("VI"=w107) -> ()  [unwired: 10 in, 1 out]
            n518 = call "Status Updated.vi"("Status"="Panel shown." ("format string")) -> ()  [unwired: 10 in, 1 out]
          }
          event User Event {
            # "Hide the panel of this VI, and send a status updated message to let listeners know."
            # "Another Module called the \"Hide Panel\" API Method."
            n519 = event-data() -> ()  [unwired: 1 in, 1 out]
            n520 = control-ref of="This VI"() -> (w109:refnum<vi>)
            n521 = call "Hide VI Panel.vi"("VI"=w109) -> ()  [unwired: 10 in, 1 out]
            n522 = call "Status Updated.vi"("Status"="Panel hidden." ("format string")) -> ()  [unwired: 10 in, 1 out]
          }
          event User Event {
            # "Another Module called the \"Get Module Execution Status\" API Method."
            n523 = event-data() -> ()  [unwired: 1 in, 1 out]
            n524 = call "Update Module Execution Status.vi"("Running?"=TRUE) -> ("error out"=w111:errorcluster)  [unwired: 10 in]
          }
          event User Event {
            # "Another Module called the \"Show Diagram\" API Method. This event is used for debugging."
            n525 = event-data() -> ()  [unwired: 1 in, 1 out]
            n526 = disable-structure shown="RUN_TIME_ENGINE==False" {
              frame condition #0 (active) {
                # "functionality not available in exe"
                n527 = invoke on="Invoke Node" class="VI" method="Lock State.Get"() -> (error out=w117:errorcluster, "Get Lock State"=w116:T8, "pwd in cache"=w113:bool)  [unwired: 4 in, 1 out]
                n528 = Equal?(x=T8."Password-protected", y=w116) -> (x = y?=w114:bool)
                n529 = Compound Arithmetic op=AND(w114, invert w113) -> (w112:bool)
                n530 = case shown="False" w112 {
                  tunnel: w117 -> [w120 _]
                  frame False {
                    n531 = property on="Property Node" class="VI"(error in=w120, "BDWin.Open"=TRUE ("Block Diagram Window:Open")) -> ()  [unwired: 1 in, 2 out]
                    n532 = call "Status Updated.vi"("Status"="Block Diagram shown." ("format string")) -> ()  [unwired: 10 in, 1 out]
                  }
                  frame True {
                    # "Password-protected VI, and the password is not in the cache. Do not show the diagram."
                  }
                }
              }
              frame condition #1 {
              }
            }
          }
          event User Event {
            # "The Stop Module Event can get fired from the Exit message in the MHL. The queue gets destroyed in that case. If the queue no longer exists, the Enqueue Exit as a priority message will return error 1. It is safe to ignore, because the module is already exiting."
            # "Another Module called the \"Stop Module\" API Method  or the Message Handling Loop below."
            n533 = event-data() -> ("Origin"=w127:string, "Exit via Stop Module Req?"=w123:bool, "Wait for Module to stop?"=w122:bool)  [unwired: 1 in]
            n534 = local write "Status"(w127) -> ()
            n535 = Bundle By Name(cluster=T9 {"Origin"="", "Exit via Stop Module Req?"=FALSE, "Wait for Module to stop?"=FALSE} ("Stop Argument"), "Exit via Stop Module Req?"=w123, "Wait for Module to stop?"=w122) -> (w121:T9)
            n536 = call-poly <vilib>:"Delacor_lib_QMH_Enqueue Message (poly).vi"("Priority Message? (F)"=TRUE, "Message Data"=w121, "Message"="Exit", "Message Queue in"=w128) -> ("error out"=w132:errorcluster)  [unwired: 6 in, 1 out]
            n537 = call <vilib>:"Clear Errors.vi"("error in (no error)"=w132, "specific error code to clear (0: all)"=1) -> ("error out"=w131:errorcluster)  [unwired: 4 in, 1 out]
          }
          event Timeout {
            n538 = event-data() -> ()  [unwired: 1 in, 3 out]
            n539 = property on="logging" class="Str"("Text.Scroll Position"=u32 99999 ("文本.滚动条位置")) -> ()  [unwired: 2 in, 2 out]
          }
          event Panel Close? {
            w137 = TRUE  # Discard the event, the MHL is responsible for closing and stopping this VI.
            # "Hide the panel or send the 'Exit' message if the user clicks the 'X' on the module main VI panel."
            n540 = event-data() -> ()  [unwired: 1 in, 1 out]
            n541 = property on="Property Node" class="Module Admin"(reference=w135) -> ("Accessors:External Launch"=w134:bool)  [unwired: 1 in, 2 out]
            n542 = case shown="True" w134 {
              tunnel: w136 -> [_ w144]
              tunnel: [_ w145] -> w138
              frame True {
                # "If externally launched, clicking the 'X' hides the panel, but doesn't close it."
                n543 = control-ref of="This VI"() -> (w141:refnum<vi>)
                n544 = call "Hide VI Panel.vi"("VI"=w141) -> ("error out"=w139:errorcluster)  [unwired: 10 in]
                n545 = call "Status Updated.vi"("error in"=w139, "Status"="Panel hidden." ("format string")) -> ()  [unwired: 9 in, 1 out]
              }
              frame False {
                # "If run as a stand-alone VI, clicking the panel 'X' stops the VI."
                n546 = call-poly <vilib>:"Delacor_lib_QMH_Enqueue Message (poly).vi"("Priority Message? (F)"=TRUE, "Message"="Exit", "Message Queue in"=w144) -> ("error out"=w145:errorcluster)  [unwired: 7 in, 1 out]
              }
            }
            n547 = event-data ("Event Filter Node")("Discard?"=w137) -> ()  [unwired: 1 in, 1 out]
          }
          event "返回主界面": Mouse Up {
            n548 = event-data() -> ()  [unwired: 1 in, 1 out]
            n549 = call-poly <vilib>:"Delacor_lib_QMH_Enqueue Message (poly).vi"("Message"="Return", "Message Queue in"=w148) -> ("error out"=w147:errorcluster)  [unwired: 8 in, 1 out]
          }
          event "任务显示": Mouse Down {
            n550 = event-data() -> ("Coords"=w157:T26)  [unwired: 1 in]
            n551 = invoke on="任务显示" class="多列列表框 (严格)" method="Point To Row Column"("Point"=w157) -> (error out=w155:errorcluster, "CellPosition"=w156:T27)  [unwired: 6 in, 5 out]
            n552 = Unbundle By Name(w156) -> ("Row"=w149:i32)
            n553 = property on="开始" class="button3 (严格)"(error in=w155) -> (error out=w152:errorcluster, "DisabledEnum"=w154:T16)  [unwired: 1 in, 1 out]
            n554 = Build Array(w149, w149) -> (w150:i32[])
            n555 = case "条件结构" shown="\"Enabled\"" w154 {
              tunnel: w153 -> [w162 _]
              tunnel: w152 -> [w161 w163]
              tunnel: [w159 w163] -> w151
              tunnel: w150 -> [w158 _]
              frame "Enabled" {
                n556 = call-poly <vilib>:"Delacor_lib_QMH_Enqueue Message (poly).vi"("error in"=w161, "Message Data Array"=w158, "Message Array"=string[] ["Select", "Show"] ("Message"), "Message Queue in"=w162) -> ("error out"=w159:errorcluster)  [unwired: 6 in, 1 out]
              }
              frame "Disabled", Default {
              }
            }
          }
          event "任务显示": Shortcut Menu Selection (User) {
            n557 = event-data() -> ("Coords"=w167:T26, "ItemTag"=w169:string)  [unwired: 1 in, 1 out]
            n558 = invoke on="任务显示" class="多列列表框 (严格)" method="Point To Row Column"("Point"=w167) -> (error out=w166:errorcluster, "CellPosition"=w165:T27)  [unwired: 6 in, 5 out]
            n559 = Unbundle By Name(w165) -> ("Row"=w164:i32)
            n560 = call-poly <vilib>:"Delacor_lib_QMH_Enqueue Message (poly).vi"("error in"=w166, "Message Data"=w164, "Message"=w169, "Message Queue in"=w170) -> ("error out"=w168:errorcluster)  [unwired: 6 in, 1 out]
          }
          event "编辑显示总览": Mouse Down {
            n561 = event-data() -> ("Coords"=w182:T26, "CtlRef"=w177:refnum<vi>)  [unwired: 1 in]
            n562 = invoke on="编辑显示总览" class="多列列表框 (严格)" method="Point To Row Column"("Point"=w182) -> ("CellPosition"=w171:T27)  [unwired: 6 in, 6 out]
            n563 = Bundle By Name(cluster=T10 {"单元格位置"={"Row"=0, "Column"=0}, "控件引用"=refnum, "进退自如"=0}, "单元格位置"=w171, "控件引用"=w177) -> (w176:T10)
            n564 = local read "Edit?"() -> (w179:bool)
            n565 = case "条件结构" shown="False" w179 {
              tunnel: w175 -> [w183 w188]
              tunnel: [_ w187] -> w174
              tunnel: w176 -> [_ w185]
              tunnel: [w183 w184] -> w172
              frame False {
              }
              frame True {
                n566 = call-poly <vilib>:"Delacor_lib_QMH_Enqueue Message (poly).vi"("Message Data"=w185, "Message"="Edit-A", "Message Queue in"=w188) -> ("error out"=w187:errorcluster, "Message Queue out"=w184:refnum<class "Delacor_lib_QMH_Message Queue.lvclass">)  [unwired: 7 in]
              }
            }
            n567 = Unbundle By Name(w171) -> ("Row"=w181:i32)
            n568 = call-poly <vilib>:"Delacor_lib_QMH_Enqueue Message (poly).vi"("error in"=w174, "Message Data"=w181, "Message"="Choose_Edit", "Message Queue in"=w172) -> ("error out"=w173:errorcluster)  [unwired: 6 in, 1 out]
          }
          event "编辑显示总览": Shortcut Menu Selection (User) {
            n569 = event-data() -> ("Coords"=w192:T26, "ItemTag"=w190:string)  [unwired: 1 in]
            n570 = invoke on="编辑显示总览" class="多列列表框 (严格)" method="Point To Row Column"("Point"=w192) -> (error out=w195:errorcluster, "CellPosition"=w194:T27)  [unwired: 6 in, 5 out]
            n571 = Unbundle By Name(w194) -> ("Row"=w193:i32)
            n572 = call-poly <vilib>:"Delacor_lib_QMH_Enqueue Message (poly).vi"("error in"=w195, "Message Data"=w193, "Message"=w190, "Message Queue in"=w191) -> ("error out"=w189:errorcluster)  [unwired: 6 in, 1 out]
          }
          event "编辑显示进表": Mouse Down {
            n573 = event-data() -> ("Coords"=w198:T26, "CtlRef"=w197:refnum<vi>)  [unwired: 1 in]
            n574 = invoke on="编辑显示进表" class="多列列表框 (严格)" method="Point To Row Column"("Point"=w198) -> ("CellPosition"=w199:T27)  [unwired: 6 in, 6 out]
            n575 = case "条件结构" shown="True" "Edit?" {
              tunnel: w201 -> [_ w209]
              tunnel: [_ w208] -> w200
              tunnel: w199 -> [_ w204]
              tunnel: w197 -> [_ w203]
              frame False {
              }
              frame True {
                n576 = Bundle By Name(cluster=T10 {"单元格位置"={"Row"=0, "Column"=0}, "控件引用"=refnum, "进退自如"=0}, "单元格位置"=w204, "控件引用"=w203, "进退自如"=u8 1) -> (w205:T10)
                n577 = call-poly <vilib>:"Delacor_lib_QMH_Enqueue Message (poly).vi"("Message Data"=w205, "Message"="Edit-1/2", "Message Queue in"=w209) -> ("error out"=w208:errorcluster)  [unwired: 7 in, 1 out]
              }
            }
          }
          event "编辑显示进表": Shortcut Menu Selection (User) {
            n578 = event-data() -> ("Coords"=w215:T26, "ItemTag"=w217:string)  [unwired: 1 in, 2 out]
            n579 = invoke on="编辑显示进表" class="多列列表框 (严格)" method="Point To Row Column"("Point"=w215) -> (error out=w214:errorcluster, "CellPosition"=w213:T27)  [unwired: 6 in, 5 out]
            n580 = Unbundle By Name(w213) -> ("Row"=w210:i32)
            n581 = Bundle By Name(cluster=cluster{"Row":i32, "进退自如":i32} {"Row"=0, "进退自如"=1}, "Row"=w210) -> (w211:cluster{"Row":i32, "进退自如":i32})
            n582 = call-poly <vilib>:"Delacor_lib_QMH_Enqueue Message (poly).vi"("error in"=w214, "Message Data"=w211, "Message"=w217, "Message Queue in"=w218) -> ("error out"=w216:errorcluster)  [unwired: 6 in, 1 out]
          }
          event "编辑显示退表": Mouse Down {
            n583 = event-data() -> ("Coords"=w222:T26, "CtlRef"=w220:refnum<vi>)  [unwired: 1 in]
            n584 = invoke on="编辑显示退表" class="多列列表框 (严格)" method="Point To Row Column"("Point"=w222) -> ("CellPosition"=w223:T27)  [unwired: 6 in, 6 out]
            n585 = local read "Edit?"() -> (w219:bool)
            n586 = case "条件结构" shown="True" w219 {
              tunnel: w221 -> [_ w231]
              tunnel: [_ w230] -> _
              tunnel: w223 -> [_ w226]
              tunnel: w220 -> [_ w225]
              frame False {
              }
              frame True {
                n587 = Bundle By Name(cluster=T10 {"单元格位置"={"Row"=0, "Column"=0}, "控件引用"=refnum, "进退自如"=0}, "单元格位置"=w226, "控件引用"=w225, "进退自如"=u8 2) -> (w227:T10)
                n588 = call-poly <vilib>:"Delacor_lib_QMH_Enqueue Message (poly).vi"("Message Data"=w227, "Message"="Edit-1/2", "Message Queue in"=w231) -> ("error out"=w230:errorcluster)  [unwired: 7 in, 1 out]
              }
            }
          }
          event "编辑显示退表": Shortcut Menu Selection (User) {
            n589 = event-data() -> ("Coords"=w237:T26, "ItemTag"=w236:string)  [unwired: 1 in]
            n590 = invoke on="编辑显示退表" class="多列列表框 (严格)" method="Point To Row Column"("Point"=w237) -> (error out=w240:errorcluster, "CellPosition"=w239:T27)  [unwired: 6 in, 5 out]
            n591 = Unbundle By Name(w239) -> ("Row"=w234:i32)
            n592 = Bundle By Name(cluster=cluster{"Row":i32, "进退自如":i32} {"Row"=0, "进退自如"=2}, "Row"=w234) -> (w233:cluster{"Row":i32, "进退自如":i32})
            n593 = call-poly <vilib>:"Delacor_lib_QMH_Enqueue Message (poly).vi"("error in"=w240, "Message Data"=w233, "Message"=w236, "Message Queue in"=w238) -> ("error out"=w232:errorcluster)  [unwired: 6 in, 1 out]
          }
          event "Combo Box": Value Change {
            n594 = event-data() -> ("NewVal"=w241:string)  [unwired: 1 in]
            n595 = call-poly <vilib>:"Delacor_lib_QMH_Enqueue Message (poly).vi"("Message Data"=w241, "Message"="Modify", "Message Queue in"=w243) -> ()  [unwired: 7 in, 2 out]
          }
          event "Valued": Value Change {
            n596 = event-data() -> ("CtlRef"=w245:refnum<vi>, "NewVal"=w246:string)  [unwired: 1 in]
            n597 = property class="Str"(reference=w245) -> ("Left"=w244:i32)  [unwired: 1 in, 2 out]
            n598 = case "条件结构" shown="2500.." w244 {
              tunnel: ["Modify-V" ("Message") "Modify" ("Message")] -> w247
              frame ..2499, Default {
              }
              frame 2500.. {
              }
            }
            n599 = call-poly <vilib>:"Delacor_lib_QMH_Enqueue Message (poly).vi"("Message Data"=w246, "Message"=w247, "Message Queue in"=w248) -> ()  [unwired: 7 in, 2 out]
          }
          event "Edit?": Value Change {
            n600 = event-data() -> ("NewVal"=w251:bool)  [unwired: 1 in]
            n601 = case "条件结构" shown="False" w251 {
              frame False {
                n602 = property on="Combo Box" class="CmbBox"("Position"=T1 {"Left"=3500, "Top"=800} ("位置")) -> ()  [unwired: 2 in, 2 out]
                n603 = property on="Valued" class="Str"("Position"=T1 {"Left"=3000, "Top"=900} ("位置")) -> ()  [unwired: 2 in, 2 out]
              }
              frame True {
              }
            }
          }
          event "开始": Value Change {
            n604 = event-data() -> ()  [unwired: 1 in, 5 out]
            n605 = call-poly <vilib>:"Delacor_lib_QMH_Enqueue Message (poly).vi"("Message"="Parse task", "Message Queue in"=w256) -> ("error out"=w255:errorcluster)  [unwired: 8 in, 1 out]
          }
          event "暂停": Value Change {
            n606 = event-data() -> ("NewVal"=w257:bool)  [unwired: 1 in]
            n607 = case "条件结构" shown="True" w257 {
              tunnel: w259 -> [w266 _]
              tunnel: [w261 w267] -> w258
              frame False {
                n608 = call-poly <vilib>:"Delacor_lib_QMH_Enqueue Message (poly).vi"("Message Data"="" ("Message"), "Message"="Pause", "Message Queue in"=w266) -> ("error out"=w265:errorcluster)  [unwired: 7 in, 1 out]
                n609 = property on="暂停" class="button3 (严格)"("布尔文本"="暂停") -> (error out=w260:errorcluster)  [unwired: 2 in, 1 out]
                n610 = Merge Errors(w260, w265) -> (w261:errorcluster)
              }
              frame True {
                n611 = property on="暂停" class="button3 (严格)"("布尔文本"="继续") -> (error out=w267:errorcluster)  [unwired: 2 in, 1 out]
              }
            }
          }
          event "结束": Value Change {
            n612 = event-data() -> ()  [unwired: 1 in, 1 out]
            n613 = call-poly <vilib>:"Delacor_lib_QMH_Enqueue Message (poly).vi"("Message"="Stop", "Message Queue in"=w269) -> ("error out"=w270:errorcluster)  [unwired: 8 in, 1 out]
          }
          event User Event {
            # "Another Module called the \"Origin\" API Method."
            n614 = event-data() -> ("原点"=w273:cluster{"Horizontal":i16, "Vertical":i16})  [unwired: 1 in]
            n615 = Bundle(cluster=T11 {"原点"={"Horizontal"=0, "Vertical"=0}} ("Origin Argument"), "原点"=w273) -> (w274:T11)
            n616 = call-poly <vilib>:"Delacor_lib_QMH_Enqueue Message (poly).vi"("Message Data"=w274, "Message"="Origin", "Message Queue in"=w277) -> ("error out"=w272:errorcluster)  [unwired: 7 in, 1 out]
          }
          event User Event {
            # "Another Module called the \"Init-External\" API Method."
            n617 = event-data() -> ("布尔"=w282:bool)  [unwired: 1 in]
            n618 = Bundle(cluster=T12 {"布尔"=FALSE} ("Init-External Argument"), "布尔"=w282) -> (w278:T12)
            n619 = call-poly <vilib>:"Delacor_lib_QMH_Enqueue Message (poly).vi"("Message Data"=w278, "Message"="逗你玩", "Message Queue in"=w279) -> ("error out"=w280:errorcluster)  [unwired: 7 in, 1 out]
          }
          event User Event {
            # "Another Module called the \"Requst Execution Status\" API Method."
            n620 = event-data() -> ("Wait Notifier"=w286:refnum<notifier>, "wait for reply"=w285:bool)  [unwired: 1 in]
            n621 = Bundle(cluster=T13 {"Wait Notifier"=refnum, "wait for reply"=FALSE} ("Requst Execution Status Argument"), "Wait Notifier"=w286, "wait for reply"=w285) -> (w287:T13)
            n622 = call-poly <vilib>:"Delacor_lib_QMH_Enqueue Message (poly).vi"("Message Data"=w287, "Message"="Requst Execution Status", "Message Queue in"=w290) -> ("error out"=w284:errorcluster)  [unwired: 7 in, 1 out]
          }
          event User Event {
            # "Another Module called the \"Receive end\" API Method."
            n623 = event-data() -> ("Arr"=w292:string[])  [unwired: 1 in]
            n624 = Bundle(cluster=T14 {"Arr"=[]} ("Receive end Argument"), "Arr"=w292) -> (w293:T14)
            n625 = call-poly <vilib>:"Delacor_lib_QMH_Enqueue Message (poly).vi"("Message Data"=w293, "Message"="Receive end", "Message Queue in"=w296) -> ("error out"=w291:errorcluster)  [unwired: 7 in, 1 out]
          }
        }
        n626 = call-dynamic "Delacor_lib_QMH_Error Handler - Event Handling Loop.vi"("error in"=w61, "Message Queue in"=w55) -> ("dup error in"=w60:errorcluster)  [unwired: 8 in, 1 out]
      }
      n627 = Unregister For Events(event registration refnum=w29) -> ()  [unwired: 1 in, 1 out]
    }
    frame Error {
      # "Synchronize Caller Events.vi will inform Start Module.vi that the module has launched and will let the code calling Start Module.vi register for broadcasts and would permit the caller receive the broadcast that an error occurred at launch time."
      n628 = call-dynamic "Delacor_lib_QMH_Release Message Queue.vi"("error in"=w1372, "Message Queue"=w1365) -> ("error out"=w1371:errorcluster)  [unwired: 9 in]
      n629 = call "Synchronize Caller Events.vi"("Singleton Module Admin in"=w1366) -> ("error out"=w1373:errorcluster)  [unwired: 9 in, 1 out]
      n630 = call "Module Name--constant.vi"() -> ("Module Name"=w1369:string)  [unwired: 11 in]
      n631 = Format Into String(format string="An error occurred during initialization. %s is no longer running.", w1369) -> (resulting string=w1367:string)  [unwired: 2 in, 1 out]
      n632 = Merge Errors(w1371, w1373) -> (w1374:errorcluster)
      n633 = call "Error Reported.vi"("Additional Information"=w1367, "Error"=w1374) -> ()  [unwired: 9 in, 1 out]
    }
  }
  n634 = Merge Errors(w2, w26) -> (w23:errorcluster)
  n635 = call "Close Module.vi"("error in"=w23, "Module Admin in"=w18) -> ("error out"=w24:errorcluster, "External Launch"=w12:bool, "Module Admin out"=w13:refnum<class "Delacor_lib_QMH_Module Admin.lvclass">)  [unwired: 7 in]
  n636 = Unregister For Events(event registration refnum=w17, error in=w24) -> (error out=w22:errorcluster)
  "error out" <- w22
  n637 = case "External Launch?" shown="True" w12 {
    tunnel: w22 -> [_ w1375]
    frame False {
    }
    frame True {
      n638 = case shown="无错误" w1375 {
        frame No Error {
          n639 = invoke on="Invoke Node" class="VI" method="FP.Close"() -> ()  [unwired: 3 in, 3 out]
        }
        frame Error {
          n640 = disable-structure shown="Default" {
            frame condition #0 (active) {
              n641 = invoke class="VI" method="FP.Open"("Activate"=TRUE ("Activate?")) -> ()  [unwired: 4 in, 5 out]
            }
            frame condition #1 {
              # "Don't show panel on error if running inside a built EXE."
            }
          }
        }
      }
    }
  }
  n642 = local write "Module Admin"(w13) -> ()
  n643 = invoke on="开始" class="button3 (严格)" method="关闭Helper Loop.vi"(error in=w2) -> ()  [unwired: 2 in, 3 out]
  n644 = invoke on="暂停" class="button3 (严格)" method="关闭Helper Loop.vi"(error in=w2) -> ()  [unwired: 2 in, 3 out]
  n645 = invoke on="结束" class="button3 (严格)" method="关闭Helper Loop.vi"(error in=w2) -> ()  [unwired: 2 in, 3 out]
  n646 = invoke on="返回主界面" class="button3 (严格)" method="关闭Helper Loop.vi"(error in=w2) -> ()  [unwired: 2 in, 3 out]
